vi "G#Debugger_GUI.vi"() -> ()   [LabVIEW 2017, in "G#Debugger.lvlib"]
doc: "Debugger for G# Objects."
uses:
  <vilib>/addons/_AddQ/G#Debugger/G#Debugger.lvlib
  <vilib>/addons/_AddQ/G#Object/G#Object.lvclass
  <vilib>/addons/_AddQ/G#Debugger/private/G#Debugger_DebugDialog.vi
  <vilib>/Platform/browser.llb/Open URL in Default Browser (string).vi
  <vilib>/addons/_AddQ/G#Debugger/G#Debugger_CloneUI.vi
  <vilib>/addons/_AddQ/G#Debugger/G#RemoteProxy/G#RemoteProxy.lvclass
panel:
  in  "OpClnUI":bool
  in  "RootClass":i32(ring) caption="G# Clone"
  in  "AggregatorsTags":i32(listbox)
  in  "Help":bool
  out "Application Instance":string
  in  "Window Behaviour":bool
  in  "Window Transparency":u8(slide) max=75 scale=0.0..75.0
  in  "External Create Process Running":bool
  in  "Tab Control":enum32{"Objects", "Trace", "Active Debug"}(tab)
  in  "Aggregators":i32(listbox)
  in  "AggregatesTags":i32(listbox)
  in  "Sorting":enum16{"Creation order", "By aggregation"}(ring)
  in  "Aggregates":i32(listbox)
  in  "Highlight Aggregates?":bool=TRUE
  out "To String":string
  in  "Attributes":bool
  in  "Inheritance":i32(listbox)
  in  "Destroy":bool
  in  "Object Tree":string(tree)
  in  "Refresh":bool
  out "# of Users":i32
  out "Counter":bool
  out "Ref Valid":bool
  out "Object Name":string
  out "Full Class Name":string
  in  "Poll Time (ms)":i32=200 min=0
  in  "Garbage collect":bool
  out "Object ID":u32 format="%x"
  in  "Hide Empty Classes?":bool=TRUE
  out "Owner":string
  in  "Connect":bool
  out "Connected?":bool
  in  "ShowAggregators":bool
  in  "Filter Expression":string
  in  "Trace Direction":bool=TRUE
  in  "Clear":bool
  in  "Save":bool
  out "Trace":string
  in  "Max Lines":u32=1000
  out "Run State":string
  out "CachedObjId":u32 caption="Object ID" format="%x"
  in  "Abort VI":bool
  in  "Run VI":bool
  in  "Open Panel":bool
  in  "DebugTree":string(tree)
  in  "Enable Active Debug":bool
  out "Icon":picture
  out "Cached Ref Valid":bool
  in  "Wait Until Done":bool=TRUE
  out "Cached Reference Class Name":string
  out "G# Version":string
  # "G# Debugger"
  # "These logs will also always appear in the NI LabVIEW Desktop Execution Trace, even without debugger running."
  # "The last created reference is automatically cashed and copied to all the new selected , opened or executed methods 'reference in'."
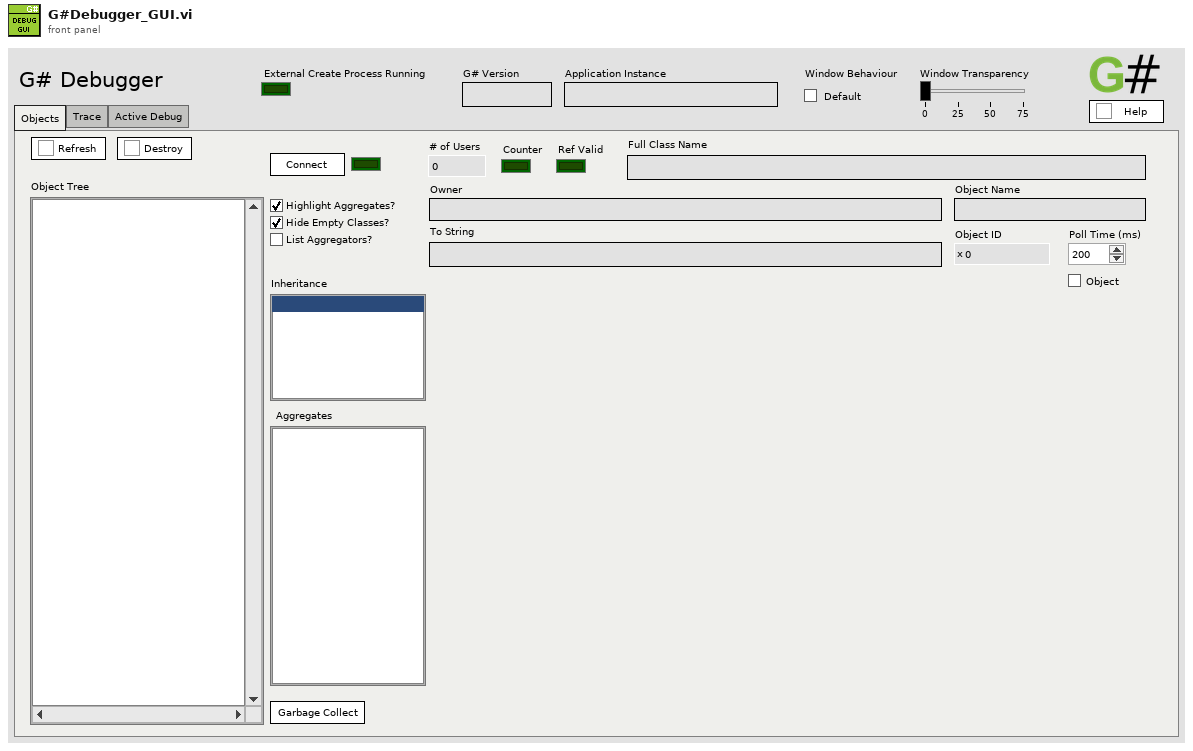
[diagram p1: front panel]
types:
  T1 = typedef "G#Debugger.lvlib/G#Debugger_Refs.ctl" = cluster{"class information dvr":refnum<data-value>, "sub panel dvr":refnum<data-value>, "GUI event":refnum<user-event>, "Active Project":refnum<vi>, "Front Panel":refnum<vi>}
  T2 = enum8{"Enabled", "Disabled", "Disabled and Grayed Out"}
  T3 = cluster{"Active Item Row Number":i32, "name":string}
  T4 = enum32{"Invalid", "Default", "Floating", "Floating/Auto-Hide", "Modal"}
  T5 = typedef "G#Debugger.lvlib/G#Debugger_SubPanelInfo.ctl" = cluster{"Ref":refnum<class "G#Object.lvclass">, "class hierarchy":T6[], "class attributes":path[], "object attributes":path[], "inheritance index":i32, "is class attributes":bool, "vi reference":refnum<vi>}
  T6 = typedef "G#Object.lvclass/G#Object_ClassHierarchy.ctl" = cluster{"ClassName":string, "FullClassName":string, "ClassPath":path, "IsLeaf":bool}
  T7 = enum32{"Bad", "Idle", "Run top level", "Running"}
  T8 = cluster{"Active Item Row Number":i32, "name":string}[]
  T9 = typedef "imagedata.ctl" = cluster{"image type":i32, "image depth":i32, "image":u8[], "mask":u8[], "colors":u32[], "Rectangle":cluster{"left":i16, "top":i16, "right":i16, "bottom":i16}}
  T10 = typedef "G#Object.lvclass/G#Object_EventType.ctl" = enum16{"Created new", "Looked up existing", "Deleted", "Forced delete", "Not deleted", "Garbage collected", "Cleared", "User", "Error", "External create object", "External create class attributes", "Created class attributes", "Run constructor", "Run constructor done", "Run open method", "Run open method done"}
  T11 = typedef "G#Object.lvclass/G#Object_ObjectInfoType.ctl" = cluster{"ObjectName":string, "ObjectID":u32, "Users":i32, "Counter":bool, "AttributeRefs":u32[], "FullClassName":string, "ClassName":string, "CreateMethod":T12, "GenericDestructorExists":bool, "Owner":string}
  T12 = typedef "G#Object.lvclass/G#Object_CreateMethod.ctl" = enum16{"Create", "Create or look up existing", "Look up existing"}
  T13 = typedef "G#Debugger.lvlib/G#Debugger_TreeElement.ctl" = cluster{"Name":string, "Tag":string, "ParentTag":string, "Position":i32}
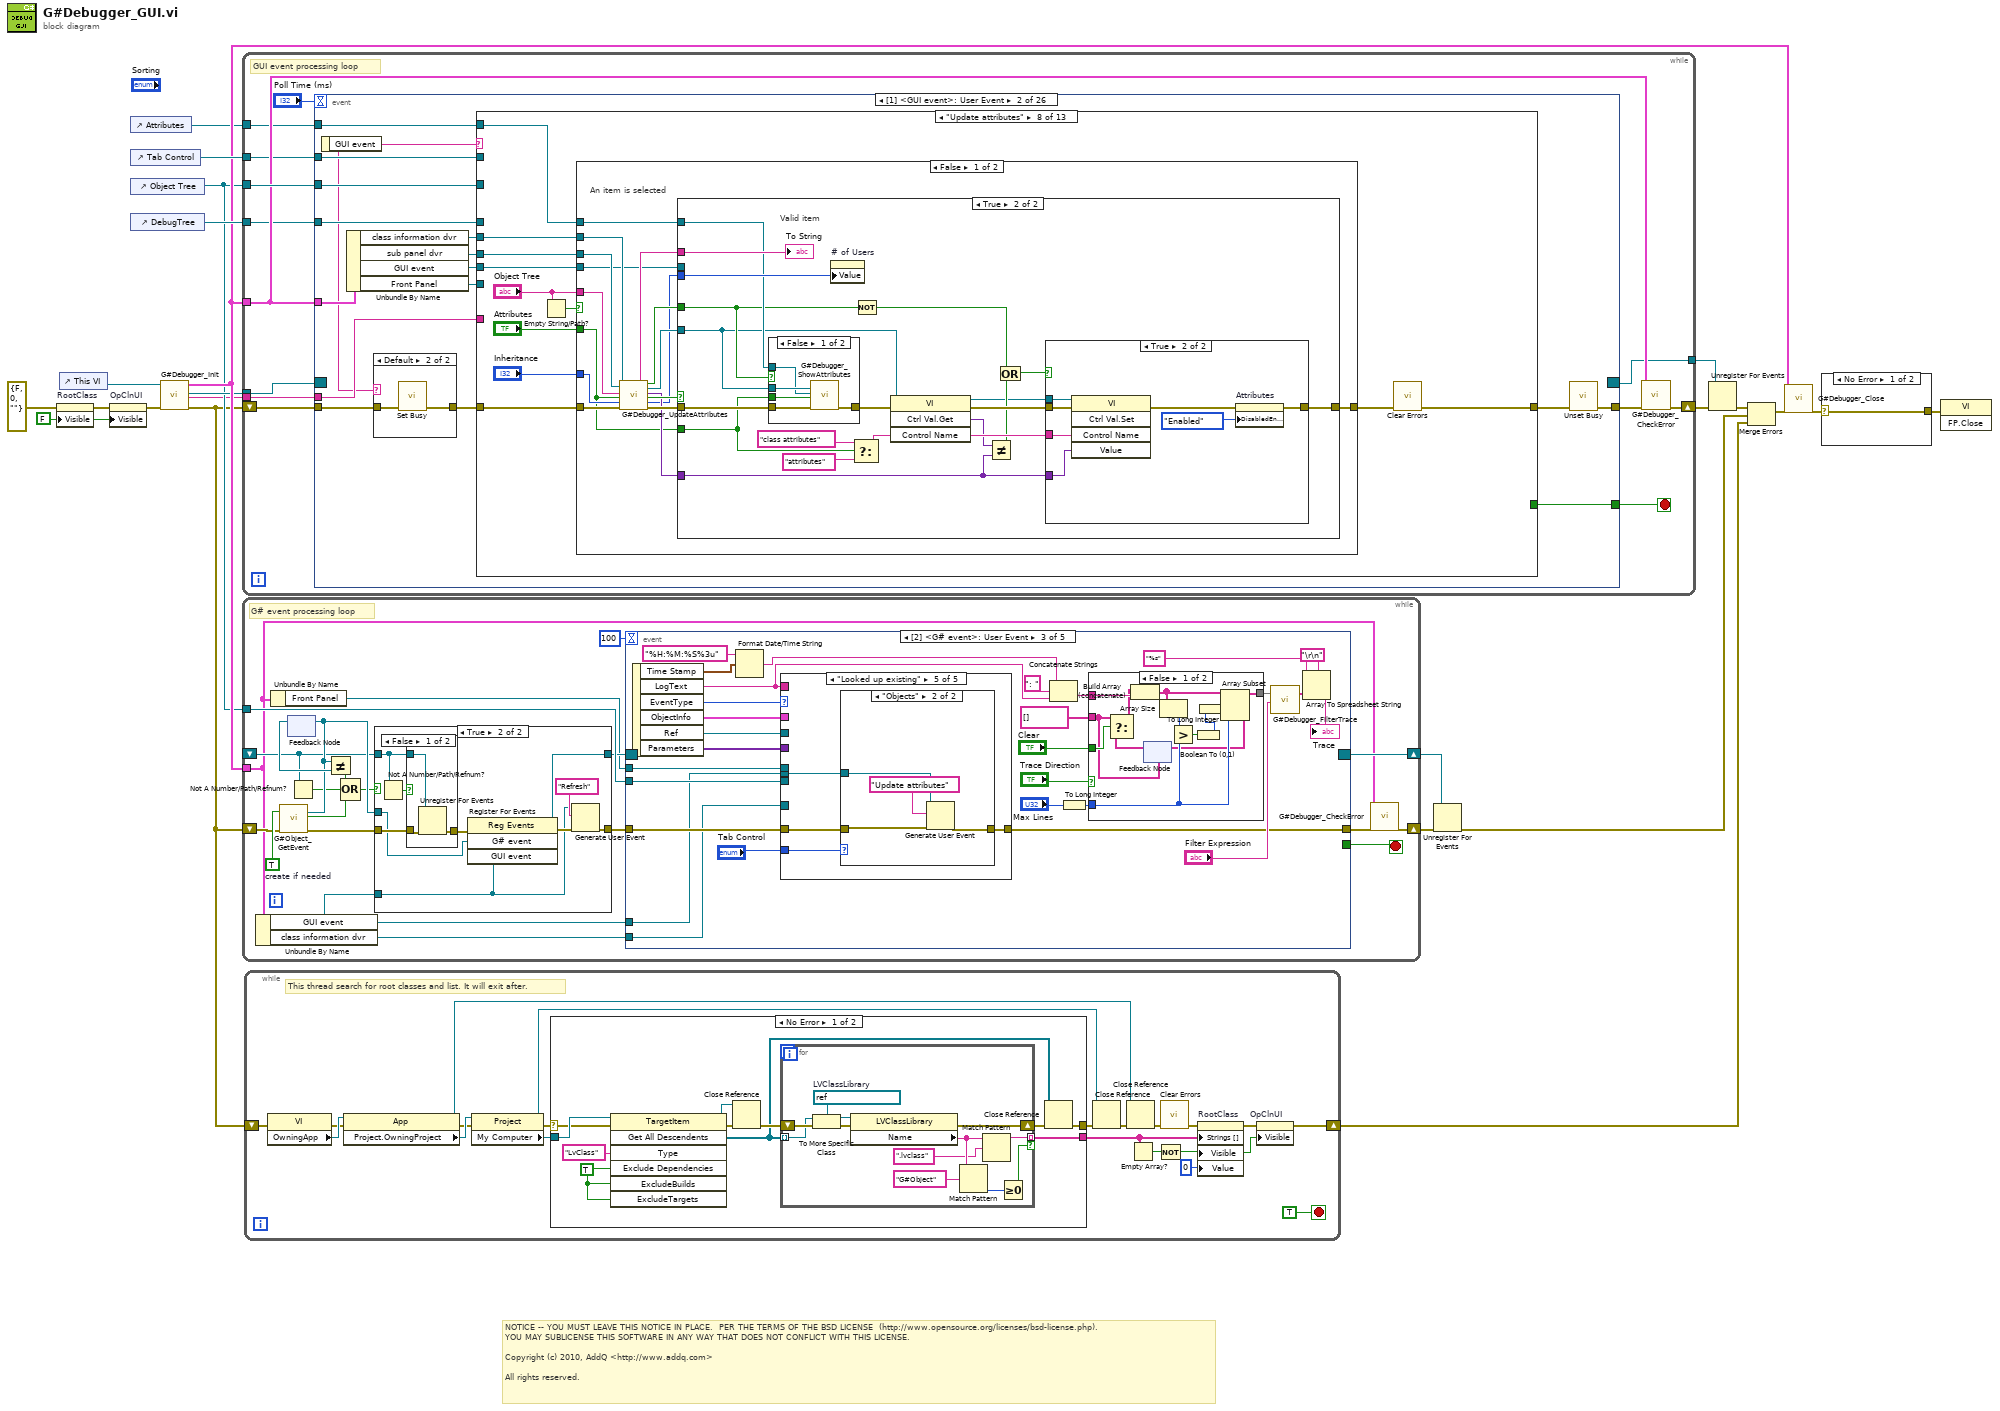
[diagram p0: block diagram]
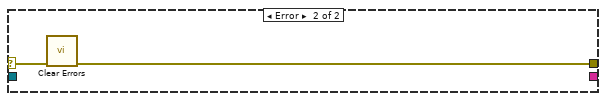
[diagram p2: hidden frame]
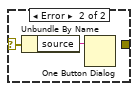
[diagram p3: hidden frame]
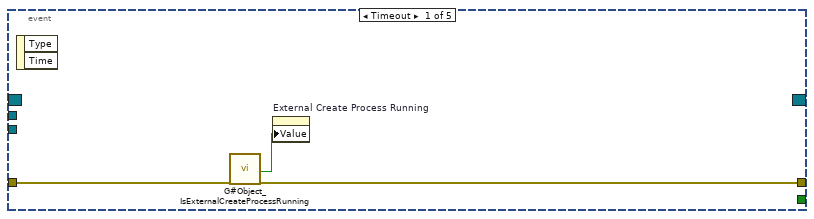
[diagram p6: hidden frame]
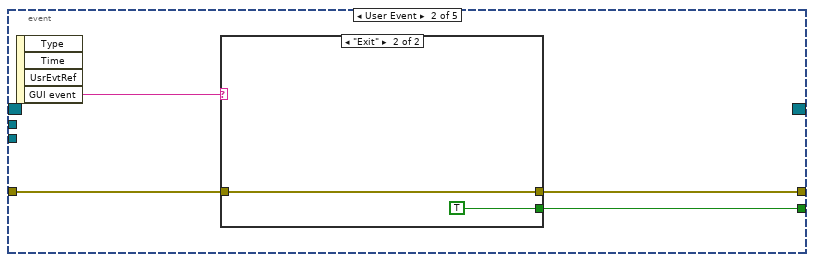
[diagram p7: hidden frame]
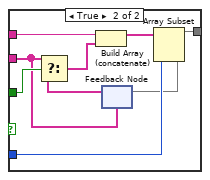
[diagram p9: hidden frame]
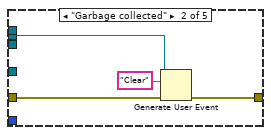
[diagram p11: hidden frame]
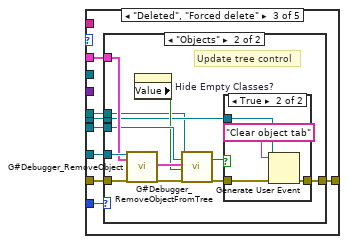
[diagram p12: hidden frame]
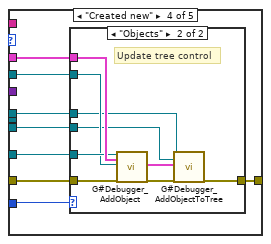
[diagram p15: hidden frame]
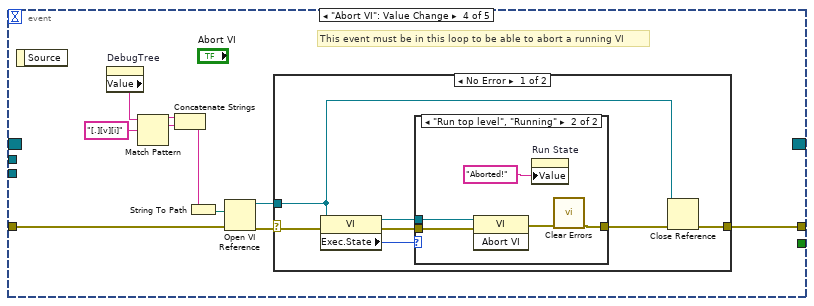
[diagram p18: hidden frame]
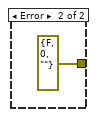
[diagram p20: hidden frame]
diagram:
  w4 = FALSE ("Visible")
  # "NOTICE -- YOU MUST LEAVE THIS NOTICE IN PLACE.  PER THE TERMS OF THE BSD LICENSE  (http://www.opensource.org/licenses/bsd-license.php).\nYOU MAY SUBLICENSE THIS SOFTWARE IN ANY WAY THAT DOES NOT CONFLICT WITH THIS LICENSE.\n\nCopyright (c) 2010, AddQ <http://www.addq.com>\n\nAll rights reserved."
  n1 = property on="RootClass" class="Ring (strict)"(error in=errorcluster {"status"=FALSE, "code"=0, "source"=""} ("error in (no error)"), "Visible"=w4) -> (error out=w3:errorcluster)  [unwired: 1 in, 1 out]
  n2 = control-ref of="This VI"() -> (w10:refnum<vi>)
  n3 = property on="OpClnUI" class="Bool"(error in=w3, "Visible"=w4) -> (error out=w1:errorcluster)  [unwired: 1 in, 1 out]
  n4 = control-ref of="Attributes"() -> (w9:refnum<vi>)
  n5 = control-ref of="Tab Control"() -> (w23:refnum<vi>)
  n6 = control-ref of="Object Tree"() -> (w12:refnum<vi>)
  n7 = control-ref of="DebugTree"() -> (w22:refnum<vi>)
  n8 = call <vilib>:"G#Debugger_Init.vi"("This VI"=w10, "error in (no error)"=w1) -> ("refs"=w21:T1, "GUI Event Registration Refnum"=w19:refnum<event-registration>, "Application Instance"=w11:string, "error out"=w6:errorcluster)  [unwired: 14 in]
  n9 = while {
    shift-right: [w34] -> w18
    shift-left: w6 -> [w29]
    tunnel: w12 -> [w36]
    tunnel: w21 -> [w32]
    tunnel: w23 -> [w31]
    tunnel: w22 -> [w30]
    tunnel: w19 -> [w28]
    tunnel: [w25] -> w17
    tunnel: w11 -> [w26]
    tunnel: w9 -> [w24]
    stop <- w35 stop-if-true
    # "GUI event processing loop"
    n10 = event shown="[1] <GUI event>: User Event" {
      selector: w28 -> [_ _ _ _ _ _ _ _ _ _ _ _ _ _ _ _ _ _ _ _ _ _ _ _ _ _]
      dyn-events: [_ _ _ _ _ _ _ _ _ _ _ _ _ _ _ _ _ _ _ _ _ _ _ _ _ _] -> w25
      timeout: "Poll Time (ms)" -> [_ _ _ _ _ _ _ _ _ _ _ _ _ _ _ _ _ _ _ _ _ _ _ _ _ _]
      tunnel: w29 -> [w42 w76 w477 w484 w494 w508 w512 w554 w589 w610 w617 w621 w628 w633 w636 w658 w683 w691 w730 w737 w740 w747 w762 w767 w788 w813]
      tunnel: [w39 w78 w477 w484 w493 w507 w511 w536 w588 w609 w618 w619 w626 w630 w640 w653 w680 w690 w729 w736 w739 w747 w761 w764 w784 w798] -> w33
      tunnel: w36 -> [_ w89 w478 w485 _ _ _ w553 _ _ w616 _ _ _ _ w652 _ _ _ _ _ _ _ w766 _ _]
      tunnel: [_ w88 _ _ _ FALSE _ _ _ _ _ _ _ _ _ _ _ _ _ _ _ _ _ _ _ _] -> w35
      tunnel: w32 -> [w46 w87 _ _ w492 w506 w510 w549 _ w608 _ w620 w627 _ w638 w649 _ w689 _ _ _ _ _ w763 _ _]
      tunnel: w31 -> [_ w84 _ _ _ _ _ _ _ _ _ _ _ _ _ _ _ _ _ _ _ _ _ _ _ _]
      tunnel: w30 -> [_ w82 _ _ _ _ _ _ _ _ _ _ _ _ _ _ _ w692 _ _ _ _ _ _ _ _]
      tunnel: w26 -> [_ w81 _ _ _ _ _ _ _ _ _ _ _ _ _ _ _ w688 _ _ _ _ _ _ _ _]
      tunnel: w24 -> [_ w74 _ _ _ _ _ _ _ _ _ _ _ _ _ _ _ _ _ _ _ _ _ _ _ _]
      event Timeout {
        # "redraw FP"
        n11 = event-data() -> ()  [unwired: 1 in, 2 out]
        n12 = Unbundle By Name(w46) -> ("Front Panel"=w40:refnum<vi>, "GUI event"=w45:refnum<user-event>)
        n13 = property on="Tab Control" class="TabCtl (strict)"(error in=w42) -> (error out=w43:errorcluster, "Value"=w44:enum32{"Objects", "Trace", "Active Debug"})  [unwired: 1 in, 1 out]
        n14 = case shown="\"Objects\"" w44 {
          tunnel: w43 -> [w47 w57 w71]
          tunnel: w45 -> [_ w53 _]
          tunnel: [w47 w54 w70] -> w41
          frame Default {
          }
          frame "Objects" {
            # "Check for dead objects, every\n5th timeout."
            n15 = Generate User Event(user event=w53, event data cluster="Update attributes" ("event data"), error in=w57) -> (error out=w55:errorcluster)  [unwired: 1 in, 1 out]
            n16 = feedback #1(u64 0) -> (w49:u64)
            n17 = Quotient & Remainder(x=w49, y=u64 5) -> (x-y*floor(x/y)=w52:u64)  [unwired: 1 out]
            n18 = Increment(x=w49) -> (x+1=w48:u64)
            n19 = feedback-in #1(w48) -> ()
            n20 = case shown="0" w52 {
              tunnel: w55 -> [w58 w63]
              tunnel: [w58 w62] -> w54
              tunnel: w53 -> [_ w61]
              frame Default {
              }
              frame 0 {
                n21 = call <vilib>:"G#Object_CleanUp.vi"("error in (no error)"=w63) -> ("any dead objects?"=w59:bool, "error out"=w60:errorcluster)  [unwired: 17 in]
                n22 = case shown="True" w59 {
                  tunnel: w60 -> [w64 w67]
                  tunnel: [w64 w66] -> w62
                  tunnel: w61 -> [_ w65]
                  frame False {
                  }
                  frame True {
                    # "Object died, refresh"
                    n23 = Generate User Event(user event=w65, event data cluster="Refresh" ("event data"), error in=w67) -> (error out=w66:errorcluster)  [unwired: 1 in, 1 out]
                  }
                }
              }
            }
          }
          frame "Active Debug" {
            w73 = FALSE  # set
            n24 = call <vilib>:"G#Debugger_CachedObject.vi"("error in (no error)"=w71, "set"=w73) -> ("not a refnum?"=w72:bool, "error out"=w70:errorcluster)  [unwired: 15 in, 1 out]
            n25 = Not(x=w72) -> (.not. x?=w69:bool)
            n26 = property on="Cached Ref Valid" class="Bool (strict)"("Value"=w69) -> ()  [unwired: 2 in, 2 out]
          }
        }
        n27 = property class="Pnl"(reference=w40, error in=w41, "DeferPanUpdts"=FALSE ("Defer Panel Updates"), "DeferPanUpdts"=TRUE ("Defer Panel Updates")) -> (error out=w39:errorcluster)  [unwired: 1 out]
      }
      event User Event {
        n28 = event-data() -> ("GUI event"=w77:string)  [unwired: 1 in]
        n29 = Unbundle By Name(w87) -> ("class information dvr"=w86:refnum<data-value>, "sub panel dvr"=w85:refnum<data-value>, "GUI event"=w83:refnum<user-event>, "Front Panel"=w80:refnum<vi>)
        n30 = case shown="Default" w77 {
          tunnel: w76 -> [w90 w92]
          tunnel: [w90 w91] -> w75
          frame "Clear object tab", "Update attributes" {
          }
          frame Default {
            n31 = call <vilib>:"Set Busy.vi"("error in (no error)"=w92) -> ("error out"=w91:errorcluster)  [unwired: 9 in, 1 out]
          }
        }
        n32 = case shown="\"Update attributes\"" w77 {
          selector: w77 -> [_ _ _ _ _ _ _ _ _ w320 _ _ w473]
          tunnel: [w93 w94 w128 w138 w145 w151 w175 w184 w276 w316 w326 w370 w474] -> w79
          tunnel: w75 -> [w93 w123 w129 w138 w144 w161 w179 w181 w277 w316 w331 w375 w474]
          tunnel: [_ _ _ _ TRUE _ _ _ _ _ _ _ _] -> w88
          tunnel: w86 -> [_ _ _ _ _ w159 w177 w187 _ _ w329 w373 _]
          tunnel: w89 -> [_ w116 _ _ _ w158 w178 _ _ _ w325 w369 _]
          tunnel: w85 -> [_ _ _ _ _ _ _ w186 _ _ _ _ _]
          tunnel: w84 -> [_ w124 _ _ _ _ _ _ _ _ _ _ _]
          tunnel: w83 -> [_ w121 w127 _ _ w150 w174 w185 _ _ _ _ _]
          tunnel: w82 -> [_ w117 _ _ _ _ _ _ _ _ _ _ _]
          tunnel: w81 -> [_ w112 _ _ _ _ _ _ _ _ _ _ _]
          tunnel: w80 -> [_ w98 _ _ _ w154 w172 _ _ _ w321 w365 _]
          tunnel: w74 -> [_ _ _ _ _ _ _ w182 _ _ _ _ _]
          frame Default {
          }
          frame "Init" {
            w95 = FALSE ("ShowAggregators")
            w99 = TRUE ("Highlight Aggregates?")
            n33 = call <vilib>:"G#Object_GetRootClassVersion.vi"("error in (no error)"=w123) -> ("version"=→"G# Version":string, "error out"=w105:errorcluster)  [unwired: 17 in]
            n34 = invoke on="Method VI Panel" class="SubPanel" method="Remove VI"(error in=w105) -> (error out=w104:errorcluster)  [unwired: 2 in, 2 out]
            n35 = call <vilib>:"G#Debugger_ClearTree.vi"("Front Panel"=w98, "Tree"=w116, "error in (no error)"=w104) -> ("error out"=w114:errorcluster)  [unwired: 16 in]
            n36 = Equal?(x=w112, y="Main Application Instance") -> (x = y?=w110:bool)
            n37 = call <vilib>:"G#Object_IsExternalCreateProcessRunning.vi"("error in (no error)"=w114) -> ("external create process running?"=w106:bool, "error out"=w113:errorcluster)  [unwired: 15 in, 2 out]
            n38 = Select(t=T2."Disabled and Grayed Out" ("Disabled"), s=w110, f=T2."Enabled" ("Disabled")) -> (s? t:f=w107:T2)
            n39 = property on="External Create Process Running" class="Bool (strict)"("Value"=w106) -> ()  [unwired: 2 in, 2 out]
            n40 = property class="TabCtl (strict)"(reference=w124, error in=w113, "Value"=enum32{"Objects", "Trace", "Active Debug"}."Objects") -> (error out=w120:errorcluster)  [unwired: 1 out]
            n41 = property on="Aggregators" class="LstBox (strict)"("Visible"=FALSE) -> ()  [unwired: 2 in, 2 out]
            n42 = property on="Enable Active Debug" class="Bool (strict)"(error in=w120, "Value"=FALSE ("Enable Active Debug"), "DisabledEnum"=w107) -> (error out=w103:errorcluster)  [unwired: 1 in, 1 out]
            n43 = property on="Aggregates" class="LstBox (strict)"("Number of Rows"=u32 16) -> ()  [unwired: 2 in, 2 out]
            n44 = call <vilib>:"G#Debugger_ClearTree.vi"("Front Panel"=w98, "Tree"=w117, "error in (no error)"=w103) -> ("error out"=w115:errorcluster)  [unwired: 16 in]
            n45 = Generate User Event(user event=w121, event data cluster="Clear controls" ("event data"), error in=w115) -> (user event out=w102:refnum<user-event>, error out=w101:errorcluster)  [unwired: 1 in]
            n46 = property on="Hide Empty Classes?" class="Bool (strict)"("Value"=w99) -> ()  [unwired: 2 in, 2 out]
            n47 = property on="Highlight Aggregates?" class="Bool (strict)"("Value"=w99) -> ()  [unwired: 2 in, 2 out]
            n48 = Generate User Event(user event=w102, event data cluster="Refresh" ("event data"), error in=w101) -> (error out=w94:errorcluster)  [unwired: 1 in, 1 out]
            n49 = property on="ShowAggregators" class="Bool (strict)"("Value"=w95) -> ()  [unwired: 2 in, 2 out]
            n50 = property on="RootClass" class="Ring (strict)"("Visible"=w95) -> ()  [unwired: 2 in, 2 out]
            n51 = property on="OpClnUI" class="Bool"("Visible"=w95) -> ()  [unwired: 2 in, 2 out]
            "Application Instance" <- w112
          }
          frame "Clear controls" {
            w130 = ""
            n52 = property on="Run State" class="Str"("Value"=w130) -> ()  [unwired: 2 in, 2 out]
            n53 = property on="Cached Reference Class Name" class="Str"("Value"=w130) -> ()  [unwired: 2 in, 2 out]
            n54 = call "Empty Picture"() -> ("empty picture"=w132:picture)
            n55 = property on="Cached Ref Valid" class="Bool (strict)"("Value"=FALSE ("Counter")) -> ()  [unwired: 2 in, 2 out]
            n56 = property on="Icon" class="Pict"("Value"=w132) -> ()  [unwired: 2 in, 2 out]
            n57 = property on="Trace" class="Str"("Value"=w130) -> ()  [unwired: 2 in, 2 out]
            n58 = property on="CachedObjId" class="DigNum (strict)"("Value"=u32 0 ("Object ID")) -> ()  [unwired: 2 in, 2 out]
            n59 = Generate User Event(user event=w127, event data cluster="Clear object tab" ("event data"), error in=w129) -> (error out=w128:errorcluster)  [unwired: 1 in, 1 out]
          }
          frame "Clear object tab" {
            w134 = 0 ("Top Row")
            w135 = string[] [] ("Item Names")
            w136 = -1 ("Inheritance")
            w137 = ""
            w141 = FALSE ("Counter")
            n60 = property on="Object Name" class="Str"("Value"=w137) -> ()  [unwired: 2 in, 2 out]
            n61 = property on="To String" class="Str"("Value"=w137) -> ()  [unwired: 2 in, 2 out]
            n62 = property on="Full Class Name" class="Str"("Value"=w137) -> ()  [unwired: 2 in, 2 out]
            n63 = property on="Owner" class="Str"("Value"=w137) -> ()  [unwired: 2 in, 2 out]
            n64 = property on="Counter" class="Bool (strict)"("Value"=w141) -> ()  [unwired: 2 in, 2 out]
            n65 = property on="Ref Valid" class="Bool (strict)"("Value"=w141) -> ()  [unwired: 2 in, 2 out]
            n66 = property on="# of Users" class="DigNum (strict)"("Value"=0 ("Nr of Users")) -> ()  [unwired: 2 in, 2 out]
            n67 = property on="Object ID" class="DigNum (strict)"("Value"=u32 0 ("Object ID")) -> ()  [unwired: 2 in, 2 out]
            n68 = property on="Aggregates" class="LstBox (strict)"("Value"=w136, "Item Names"=w135, "Top Row"=w134) -> ()  [unwired: 2 in, 2 out]
            n69 = property on="Inheritance" class="LstBox (strict)"("Value"=w136, "Item Names"=w135, "Top Row"=w134) -> ()  [unwired: 2 in, 2 out]
            n70 = property on="Aggregators" class="LstBox (strict)"("Value"=w136, "Item Names"=w135, "Top Row"=w134) -> ()  [unwired: 2 in, 2 out]
          }
          frame "Exit" {
            n71 = property on="Enable Active Debug" class="Bool (strict)"(error in=w144) -> (error out=w143:errorcluster, "Value"=w142:bool)  [unwired: 1 in, 1 out]
            n72 = case shown="True" w142 {
              tunnel: [w147 w149] -> w145
              tunnel: w143 -> [w147 w148]
              frame False {
              }
              frame True {
                n73 = call <vilib>:"GarbageCollector.vi"("error in (no error)"=w148) -> ("error out"=w149:errorcluster)  [unwired: 16 in, 2 out]
              }
            }
          }
          frame "Refresh" {
            # "Refresh tree list"
            n74 = call <vilib>:"G#Debugger_Refresh.vi"("Objects dvr"=w159, "error in (no error)"=w161) -> ("error out"=w160:errorcluster)  [unwired: 17 in]
            n75 = call <vilib>:"G#Debugger_PopulateObjectTree.vi"("Objects dvr"=w159, "Tree"=w158, "hide empty classes?"="Hide Empty Classes?", "error in (no error)"=w160, "Front Panel"=w154) -> ("error out"=w156:errorcluster)  [unwired: 14 in]
            n76 = property on="Highlight Aggregates?" class="Bool (strict)"() -> ("Value"=w155:bool)  [unwired: 2 in, 2 out]
            n77 = case shown="True" w155 {
              tunnel: [w167 w170] -> w152
              tunnel: w156 -> [w167 w169]
              tunnel: w150 -> [_ w168]
              frame False {
              }
              frame True {
                n78 = Generate User Event(user event=w168, event data cluster="Highlight aggregates" ("event data"), error in=w169) -> (error out=w170:errorcluster)  [unwired: 1 in, 1 out]
              }
            }
            n79 = property on="ShowAggregators" class="Bool (strict)"() -> ("Value"=w153:bool)  [unwired: 2 in, 2 out]
            n80 = case shown="True" w153 {
              tunnel: w152 -> [w162 w165]
              tunnel: [w162 w164] -> w151
              tunnel: w150 -> [_ w163]
              frame False {
              }
              frame True {
                n81 = Generate User Event(user event=w163, event data cluster="ListAggregators" ("event data"), error in=w165) -> (error out=w164:errorcluster)  [unwired: 1 in, 1 out]
              }
            }
          }
          frame "Clear" {
            # "Clears tree and object cache"
            n82 = call <vilib>:"G#Debugger_ClearTree.vi"("Front Panel"=w172, "Tree"=w178, "error in (no error)"=w179) -> ("error out"=w180:errorcluster)  [unwired: 16 in]
            n83 = call <vilib>:"G#Debugger_Clear.vi"("Objects dvr"=w177, "error in (no error)"=w180) -> ("error out"=w176:errorcluster)  [unwired: 17 in]
            n84 = Generate User Event(user event=w174, event data cluster="Clear object tab" ("event data"), error in=w176) -> (error out=w175:errorcluster)  [unwired: 1 in, 1 out]
          }
          frame "Update attributes" {
            n85 = Empty String/Path?(string/path="Object Tree") -> (empty?=w189:bool)
            n86 = case shown="False" w189 {
              tunnel: w181 -> [w207 w261]
              tunnel: w187 -> [w206 _]
              tunnel: w186 -> [w205 w259]
              tunnel: "Object Tree" -> [w204 _]
              tunnel: "Attributes" -> [w192 _]
              tunnel: "Inheritance" -> [w203 _]
              tunnel: [w200 w255] -> w183
              tunnel: w185 -> [w195 w254]
              tunnel: w182 -> [w193 _]
              frame False {
                # "An item is selected"
                n87 = call <vilib>:"G#Debugger_UpdateAttributes.vi"("Objects dvr"=w206, "Subpanel dvr"=w205, "tag"=w204, "class attributes"=w192, "inheritance index"=w203, "error in (no error)"=w207) -> ("string"=w196:string, "Only read attributes"=w199:bool, "attributes reference"=w198:refnum<vi>, "attributes value"=w197:variant, "valid object"=w202:bool, "# of users?"=w194:i32, "error out"=w201:errorcluster)  [unwired: 7 in]
                n88 = case shown="True" w202 {
                  tunnel: w201 -> [w215 w235]
                  tunnel: [w209 w236] -> w200
                  tunnel: w199 -> [_ w225]
                  tunnel: w198 -> [_ w221]
                  tunnel: w197 -> [_ w228]
                  tunnel: w196 -> [_ w238]
                  tunnel: w195 -> [w208 _]
                  tunnel: w194 -> [_ w237]
                  tunnel: w193 -> [_ w234]
                  tunnel: w192 -> [_ w231]
                  frame False {
                    # "Subpanel info is invalid->Clear"
                    n89 = invoke on="Attributes" class="SubPanel" method="Remove VI"(error in=w215) -> (error out=w214:errorcluster)  [unwired: 2 in, 2 out]
                    n90 = call <vilib>:"G#Object_CleanUp.vi"("error in (no error)"=w214) -> ("any dead objects?"=w212:bool, "error out"=w213:errorcluster)  [unwired: 17 in]
                    n91 = case shown="True" w212 {
                      tunnel: [w217 w219] -> w210
                      tunnel: w213 -> [w217 w219]
                      tunnel: ["Clear object tab" ("event data") "Refresh" ("event data")] -> w211
                      frame False {
                      }
                      frame True {
                      }
                    }
                    n92 = Generate User Event(user event=w208, event data cluster=w211, error in=w210) -> (error out=w209:errorcluster)  [unwired: 1 in, 1 out]
                  }
                  frame True {
                    # "Valid item"
                    n93 = case shown="False" w225 {
                      tunnel: w235 -> [w251 w252]
                      tunnel: w234 -> [w248 _]
                      tunnel: [w250 w252] -> w226
                      tunnel: w221 -> [w249 _]
                      tunnel: w231 -> [w247 _]
                      frame False {
                        n94 = call <vilib>:"G#Debugger_ShowAttributes.vi"("VIRef"=w249, "SubPanel"=w248, "ClassAttributes"=w247, "error in (no error)"=w251) -> ("error out"=w250:errorcluster)  [unwired: 14 in, 1 out]
                      }
                      frame True {
                      }
                    }
                    n95 = property on="# of Users" class="DigNum (strict)"("Value"=w237) -> ()  [unwired: 2 in, 2 out]
                    n96 = Select(t="class attributes" ("y"), s=w231, f="attributes" ("y")) -> (s? t:f=w230:string)
                    n97 = Not(x=w225) -> (.not. x?=w224:bool)
                    n98 = invoke class="VI" method="Ctrl Val.Get"(reference=w221, error in=w226, "Control Name"=w230) -> (reference out=w220:refnum<vi>, error out=w227:errorcluster, "Get Control Value Variant"=w229:variant)  [unwired: 1 in, 1 out]
                    n99 = Not Equal?(x=w229, y=w228) -> (x != y?=w223:bool)
                    n100 = Or(x=w224, y=w223) -> (x .or. y?=w222:bool)
                    n101 = case shown="True" w222 {
                      tunnel: [w239 w245] -> w236
                      tunnel: w227 -> [w239 w243]
                      tunnel: w220 -> [_ w242]
                      tunnel: w230 -> [_ w241]
                      tunnel: w228 -> [_ w240]
                      frame False {
                      }
                      frame True {
                        n102 = invoke class="VI" method="Ctrl Val.Set"(reference=w242, error in=w243, "Control Name"=w241, "Value"=w240) -> (error out=w246:errorcluster)  [unwired: 1 in, 4 out]
                        n103 = property on="Attributes" class="SubPnl"(error in=w246, "DisabledEnum"=T2."Enabled" ("Disabled")) -> (error out=w245:errorcluster)  [unwired: 1 in, 1 out]
                      }
                    }
                    "To String" <- w238
                  }
                }
              }
              frame True {
                # "No item selected in tree"
                n104 = invoke on="Attributes" class="SubPanel" method="Remove VI"(error in=w261) -> (error out=w260:errorcluster)  [unwired: 2 in, 2 out]
                n105 = in-place {
                  in-place-border: w260 -> [w266]
                  in-place-border: [w264] -> w257
                  # "Force a subpanel update!"
                  n106 = in-place-dvr #2(w259) -> (w265:T5)  [unwired: 1 out]
                  n107 = Unbundle By Name(w265) -> ("vi reference"=w262:refnum<vi>)
                  n108 = Not A Number/Path/Refnum?(number/path/refnum=w262) -> (NaN/Path/Refnum?=w263:bool)
                  n109 = case shown="False" w263 {
                    tunnel: w266 -> [w269 w270]
                    tunnel: [w268 w270] -> w264
                    tunnel: w262 -> [w267 _]
                    frame False {
                      n110 = Close Reference(reference=w267, error in (no error)=w269) -> (error out=w268:errorcluster)
                    }
                    frame True {
                    }
                  }
                  n111 = in-place-dvr #2(w265) -> (w258:errorcluster)  [unwired: 1 out]
                }
                n112 = Merge Errors(w258, w257) -> (w256:errorcluster)
                n113 = Generate User Event(user event=w254, event data cluster="Clear object tab" ("event data"), error in=w256) -> (error out=w255:errorcluster)  [unwired: 1 in, 1 out]
              }
            }
            n114 = call <vilib>:"Clear Errors.vi"("error in (no error)"=w183) -> ("error out"=w184:errorcluster)  [unwired: 5 in, 1 out]
          }
          frame "Run VI" {
            n115 = property on="DebugTree" class="Tree (strict)"() -> ("Value"=w271:string)  [unwired: 2 in, 2 out]
            n116 = Match Pattern(string=w271, regular expression="[.][v][i]") -> (before substring=w274:string, match substring=w273:string)  [unwired: 1 in, 2 out]
            n117 = Concatenate Strings(w274, w273) -> (w272:string)
            n118 = String To Path(string=w272) -> (path=w278:path)
            n119 = Open VI Reference(vi path=w278, error in (no error)=w277) -> (vi reference=w280:refnum<vi>, error out=w279:errorcluster)  [unwired: 4 in]
            n120 = case shown="No Error" w279 {
              selector: w279 -> [w285 _]
              tunnel: [w291 errorcluster {"status"=FALSE, "code"=0, "source"=""} ("error in (no error)")] -> w276
              tunnel: w280 -> [w284 _]
              tunnel: w278 -> [w289 _]
              frame No Error {
                n121 = stacked-sequence {
                  tunnel: w289 -> [w297]
                  tunnel: [w297] -> w288
                  frame #0 {
                    "Run State" <- "Running..." ("Run State")
                  }
                }
                n122 = property class="VI"(reference=w284, error in=w285) -> (error out=w282:errorcluster, "Exec.State"=w283:T7, "Exec.IsReentrant"=w286:bool)  [unwired: 1 out]
                n123 = case shown="\"Run top level\"" w283 {
                  tunnel: [FALSE TRUE w294 w295] -> w287
                  tunnel: w286 -> [_ _ w294 w295]
                  frame Default {
                  }
                  frame "Idle" {
                  }
                  frame "Run top level" {
                  }
                  frame "Running" {
                  }
                }
                n124 = case shown="True" w287 {
                  tunnel: [w303 w311] -> w290
                  tunnel: w282 -> [w303 w306]
                  tunnel: w288 -> [w302 _]
                  tunnel: [w299 w314] -> w281
                  tunnel: w283 -> [w298 _]
                  tunnel: w284 -> [_ w307]
                  frame False {
                    n125 = Strip Path(path=w302) -> (name=w301:string)  [unwired: 1 out]
                    n126 = Format Into String(format string="%s is not reentrant or in idle execution state! (%s)", w301, w298) -> (resulting string=w299:string)  [unwired: 2 in, 1 out]
                  }
                  frame True {
                    n127 = call <vilib>:"G#Debugger_RunVI.vi"("vi reference"=w307, "wait until done"="Wait Until Done", "error in (no error)"=w306) -> ("class name"=→"Cached Reference Class Name":string, "object ID"=→"CachedObjId":u32, "message"=w310:string, "not a refnum?"=w305:bool, "error out"=w311:errorcluster)  [unwired: 12 in]
                    n128 = Not(x=w305) -> (.not. x?=→"Cached Ref Valid":bool)
                    n129 = Select(t=w310, s="Wait Until Done", f="Run state is not available!") -> (s? t:f=w314:string)
                  }
                }
                n130 = property on="Run State" class="Str"("Value"=w281) -> ()  [unwired: 2 in, 2 out]
                n131 = Close Reference(reference=w284, error in (no error)=w290) -> (error out=w291:errorcluster)
              }
              frame Error {
              }
            }
          }
          frame "Wait".."Wb" {
            n132 = Decimal String To Number(string=w320, offset=5, default (0L)=u32 0 ("default (0 I32)")) -> (number=w317:u32)  [unwired: 1 out]
            n133 = Wait (ms)(milliseconds to wait=w317) -> ()  [unwired: 1 out]
          }
          frame "Highlight aggregates" {
            n134 = property on="Property Node" class="Tree (strict)"(reference=w325, error in=w331) -> (error out=w330:errorcluster, "Value"=w328:string)  [unwired: 1 out]
            n135 = call <vilib>:"G#Debugger_GetObjectFromTag.vi"("Objects dvr"=w329, "Tag"=w328, "class attributes"=FALSE, "error in (no error)"=w330) -> ("Ref"=w324:refnum<class "G#Object.lvclass">, "Found"=w322:bool, "error out"=w323:errorcluster)  [unwired: 13 in]
            n136 = case shown="True" w322 {
              tunnel: [w332 w340] -> w326
              tunnel: w325 -> [_ w352]
              tunnel: w324 -> [_ w351]
              tunnel: w323 -> [w332 w349]
              tunnel: w321 -> [_ w339]
              frame False {
              }
              frame True {
                w346 = TRUE  # remove duplicates
                # "redraw FP"
                n137 = property on="Attributes" class="Bool (strict)"(error in=w349) -> (error out=w348:errorcluster, "Value"=w347:bool)  [unwired: 1 in, 1 out]
                n138 = call <vilib>:"G#Object_GetAggregatedObjects.vi"("reference in"=w351, "class attributes (F)"=w347, "remove duplicates (F)"=w346, "error in (no error)"=w348) -> ("aggregated objects"=w345:refnum<class "G#Object.lvclass">[], "error out"=w344:errorcluster)  [unwired: 12 in, 2 out]
                n139 = for {
                  tunnel: w345 -> [w355] mode=indexing
                  shift-right: [w356] -> w350
                  shift-left: w344 -> [w358]
                  tunnel: [w357] -> w333 mode=indexing if=w353
                  n140 = call-dynamic "NotARefNum.vi"("reference in"=w355) -> ("not a refnum?"=w354:bool)  [unwired: 1 in, 1 out]
                  n141 = case shown="False" w354 {
                    tunnel: w355 -> [w363 _]
                    tunnel: w358 -> [w362 w364]
                    tunnel: [w360 _] -> w357
                    tunnel: [w359 w364] -> w356
                    frame False {
                      # "ObjectIDs are the\ntags in the object tree"
                      n142 = call-dynamic "GetObjectID.vi"("reference in"=w363, "error in (no error)"=w362) -> ("object ID"=w361:u32, "error out"=w359:errorcluster)  [unwired: 15 in, 1 out]
                      n143 = Number To Decimal String(number=w361) -> (decimal integer string=w360:string)  [unwired: 1 in]
                    }
                    frame True {
                    }
                  }
                  n144 = Not(x=w354) -> (.not. x?=w353:bool)
                }
                n145 = control-ref of="Aggregates"() -> (w338:refnum<vi>)
                n146 = control-ref of="AggregatesTags"() -> (w337:refnum<vi>)
                n147 = Array Size(array=w333) -> (size(s)=w336:i32)
                n148 = call <vilib>:"G#Debugger_Highlight.vi"("Tree"=w352, "Aggregates"=w338, "ObjectIDs"=w333, "error in (no error)"=w350, "AggregatesTags"=w337) -> ("error out"=w341:errorcluster)  [unwired: 14 in]
                n149 = Greater Or Equal?(x=w336, y=8) -> (x >= y?=w335:bool)
                n150 = property class="Pnl"(reference=w339, error in=w341, "DeferPanUpdts"=FALSE ("Defer Panel Updates"), "DeferPanUpdts"=TRUE ("Defer Panel Updates")) -> (error out=w340:errorcluster)  [unwired: 1 out]
                n151 = property on="Aggregates" class="LstBox (strict)"("Scrollbar Visible"=w335) -> ()  [unwired: 2 in, 2 out]
              }
            }
          }
          frame "ListAggregators" {
            n152 = property on="Property Node" class="Tree (strict)"(reference=w369, error in=w375) -> (error out=w374:errorcluster, "Value"=w372:string)  [unwired: 1 out]
            n153 = call <vilib>:"G#Debugger_GetObjectFromTag.vi"("Objects dvr"=w373, "Tag"=w372, "class attributes"=FALSE, "error in (no error)"=w374) -> ("Ref"=w368:refnum<class "G#Object.lvclass">, "Found"=w366:bool, "error out"=w367:errorcluster)  [unwired: 13 in]
            n154 = case shown="True" w366 {
              tunnel: [w376 w396] -> w370
              tunnel: w369 -> [_ _]
              tunnel: w368 -> [_ w395]
              tunnel: w367 -> [w376 w401]
              tunnel: w365 -> [_ w381]
              frame False {
              }
              frame True {
                # "redraw FP"
                n155 = call-dynamic "GetObjectID.vi"("reference in"=w395) -> ("object ID"=w378:u32)  [unwired: 16 in, 2 out]
                n156 = property on="Attributes" class="Bool (strict)"(error in=w401) -> (error out=w400:errorcluster, "Value"=w399:bool)  [unwired: 1 in, 1 out]
                n157 = Equal To 0?(x=w378) -> (x = 0?=w377:bool)
                n158 = case shown="False" w377 {
                  tunnel: w400 -> [w413 w464]
                  tunnel: w399 -> [w412 _]
                  tunnel: w378 -> [w406 _]
                  tunnel: [w405 w464] -> w394
                  tunnel: [w403 _] -> w387
                  tunnel: [w402 _] -> w385
                  frame False {
                    w411 = TRUE  # remove duplicates
                    n159 = call <vilib>:"G#Object_GetAllObjects.vi"("only refs (F)"=TRUE) -> ("all refs"=w408:refnum<class "G#Object.lvclass">[])  [unwired: 15 in, 3 out]
                    n160 = for {
                      tunnel: w412 -> [w420]
                      tunnel: w411 -> [w419]
                      tunnel: [w417] -> w410 mode=indexing if=w414
                      shift-right: [w418] -> w409
                      shift-left: w413 -> [w421]
                      tunnel: w408 -> [w416] mode=indexing
                      tunnel: [w416] -> w404 mode=indexing if=w414
                      n161 = call-dynamic "NotARefNum.vi"("reference in"=w416) -> ("not a refnum?"=w415:bool)  [unwired: 1 in, 1 out]
                      n162 = Not(x=w415) -> (.not. x?=w414:bool)
                      n163 = case shown="False" w415 {
                        tunnel: w421 -> [w428 w433]
                        tunnel: w420 -> [w427 _]
                        tunnel: w419 -> [w426 _]
                        tunnel: [w425 w433] -> w418
                        tunnel: w416 -> [w424 _]
                        tunnel: [w422 _] -> w417
                        frame False {
                          n164 = call <vilib>:"G#Object_GetAggregatedObjects.vi"("reference in"=w424, "class attributes (F)"=w427, "remove duplicates (F)"=w426, "error in (no error)"=w428) -> ("aggregated objects"=w423:refnum<class "G#Object.lvclass">[], "error out"=w425:errorcluster)  [unwired: 12 in, 2 out]
                          n165 = for {
                            tunnel: w423 -> [w432] mode=indexing
                            tunnel: [w431] -> w422 mode=indexing if=w429
                            n166 = call-dynamic "NotARefNum.vi"("reference in"=w432) -> ("not a refnum?"=w430:bool, "reference out"=w431:refnum<class "G#Object.lvclass">)  [unwired: 1 in]
                            n167 = Not(x=w430) -> (.not. x?=w429:bool)
                          }
                        }
                        frame True {
                        }
                      }
                    }
                    n168 = for {
                      tunnel: w410 -> [w444] mode=indexing
                      shift-right: [w440] -> w405
                      shift-left: w409 -> [w443]
                      tunnel: [w436] -> w403 mode=indexing if=w434
                      tunnel: w406 -> [w442]
                      tunnel: w404 -> [w439] mode=indexing
                      tunnel: [w435] -> w402 mode=indexing if=w434
                      # "ObjectIDs are the\ntags in the object tree"
                      n169 = for {
                        tunnel: w444 -> [w455] mode=indexing
                        tunnel: w442 -> [w453]
                        tunnel: [w450] -> w434
                        shift-right: [w451] -> w441
                        shift-left: w443 -> [w454]
                        stop <- w450 stop-if-true
                        n170 = call-dynamic "GetObjectID.vi"("reference in"=w455, "error in (no error)"=w454) -> ("object ID"=w452:u32, "error out"=w451:errorcluster)  [unwired: 15 in, 1 out]
                        n171 = Equal?(x=w453, y=w452) -> (x = y?=w450:bool)
                      }
                      n172 = case shown="True" w434 {
                        tunnel: w441 -> [w456 w463]
                        tunnel: [w456 w462] -> w440
                        tunnel: w439 -> [_ w458]
                        tunnel: [_ w460] -> w438
                        tunnel: [_ w459] -> w437
                        tunnel: [_ w457] -> w435
                        frame False {
                        }
                        frame True {
                          n173 = call-dynamic "GetObjectID.vi"("reference in"=w458) -> ("object ID"=w457:u32)  [unwired: 16 in, 2 out]
                          n174 = call-dynamic "GetObjectStatus.vi"("reference in"=w458, "simple info (F)"=TRUE, "error in (no error)"=w463) -> ("class name"=w460:string, "object name"=w459:string, "error out"=w462:errorcluster)  [unwired: 5 in, 9 out]
                        }
                      }
                      n175 = disable-structure shown="Enabled" {
                        disable-tunnel: w438 -> [w448 _]
                        disable-tunnel: w437 -> [w447 w449]
                        disable-tunnel: [w445 w449] -> w436
                        frame Enabled {
                          n176 = Format Into String(format string="%s:%s", w448, w447) -> (resulting string=w445:string)  [unwired: 2 in, 1 out]
                        }
                        frame Disabled {
                        }
                      }
                    }
                  }
                  frame True {
                  }
                }
                n177 = for {
                  tunnel: w385 -> [w469] mode=indexing
                  tunnel: w387 -> [w470] mode=indexing
                  tunnel: [w468] -> w389 mode=indexing
                  n178 = Bundle(cluster=T3 {"Active Item Row Number"=0, "name"=""}, "Active Item Row Number"=w469, "name"=w470) -> (w468:T3)
                }
                n179 = Sort 1D Array(array=w385) -> (sorted array=w384:u32[])
                n180 = Array Size(array=w384) -> (size(s)=w392:i32)
                n181 = Greater Or Equal?(x=w392, y=7) -> (x >= y?=w391:bool)
                n182 = Number To Decimal String(number=w384) -> (decimal integer string=w382:string[])  [unwired: 1 in]
                n183 = property on="Aggregators" class="LstBox (strict)"("Scrollbar Visible"=w391) -> ()  [unwired: 2 in, 2 out]
                n184 = Sort 1D Array(array=w389) -> (sorted array=w388:T8)
                n185 = for {
                  tunnel: w388 -> [w466] mode=indexing
                  tunnel: [w465] -> w386 mode=indexing
                  n186 = Unbundle By Name(w466) -> ("name"=w465:string)
                }
                n187 = property on="Aggregators" class="LstBox (strict)"(error in=w394, "Item Names"=w386) -> (error out=w393:errorcluster)  [unwired: 1 in, 1 out]
                n188 = control-ref of="AggregatorsTags"() -> (w390:refnum<vi>)
                n189 = property on="Property Node" class="LstBox (strict)"(reference=w390, "Item Names"=w382, "Value"=-1, "Top Row"=0) -> ()  [unwired: 1 in, 2 out]
                n190 = property class="Pnl"(reference=w381, error in=w393, "DeferPanUpdts"=FALSE ("Defer Panel Updates"), "DeferPanUpdts"=TRUE ("Defer Panel Updates")) -> (error out=w396:errorcluster)  [unwired: 1 out]
              }
            }
          }
          frame "Connected", "Disconnected" {
            n191 = Equal?(x=w473, y="Connected") -> (x = y?=→"Connected?":bool)
          }
        }
        n192 = call <vilib>:"Unset Busy.vi"("error in (no error)"=w79) -> ("error out"=w78:errorcluster)  [unwired: 10 in]
      }
      event "Aggregates": Double Click {
        n193 = event-data() -> ()  [unwired: 1 in, 1 out]
        n194 = control-ref of="AggregatesTags"() -> (w476:refnum<vi>)
        n195 = control-ref of="Aggregates"() -> (w475:refnum<vi>)
        n196 = property class="LstBox (strict)"(reference=w476) -> ("Item Names"=w480:string[])  [unwired: 1 in, 2 out]
        n197 = property class="LstBox (strict)"(reference=w475) -> ("Value"=w481:i32)  [unwired: 1 in, 2 out]
        n198 = Index Array(array=w480, index=w481) -> (element=w479:string)
        n199 = property class="Tree (strict)"(reference=w478, "Val(Sgnl)"=w479) -> ()  [unwired: 1 in, 2 out]
      }
      event "Aggregators": Double Click {
        n200 = event-data() -> ()  [unwired: 1 in, 1 out]
        n201 = control-ref of="AggregatorsTags"() -> (w483:refnum<vi>)
        n202 = control-ref of="Aggregators"() -> (w482:refnum<vi>)
        n203 = property class="LstBox (strict)"(reference=w482) -> ("Value"=w488:i32)  [unwired: 1 in, 2 out]
        n204 = property class="LstBox (strict)"(reference=w483) -> ("Item Names"=w487:string[])  [unwired: 1 in, 2 out]
        n205 = Index Array(array=w487, index=w488) -> (element=w486:string)
        n206 = property class="Tree (strict)"(reference=w485, "Val(Sgnl)"=w486) -> ()  [unwired: 1 in, 2 out]
      }
      event "ShowAggregators": Value Change {
        n207 = event-data() -> ("NewVal"=w490:bool)  [unwired: 1 in]
        n208 = Unbundle By Name(w492) -> ("GUI event"=w491:refnum<user-event>)
        n209 = property on="Aggregators" class="LstBox (strict)"("Visible"=w490) -> ()  [unwired: 2 in, 2 out]
        n210 = case shown="False" w490 {
          tunnel: w494 -> [w496 w500]
          tunnel: [w496 w499] -> w493
          tunnel: w491 -> [_ w498]
          tunnel: [u32 16 ("Number of Rows") u32 7 ("Number of Rows")] -> w489
          frame False {
          }
          frame True {
            n211 = Generate User Event(user event=w498, event data cluster="ListAggregators" ("event data"), error in=w500) -> (error out=w499:errorcluster)  [unwired: 1 in, 1 out]
          }
        }
        n212 = property on="Aggregates" class="LstBox (strict)"("Number of Rows"=w489) -> ()  [unwired: 2 in, 2 out]
      }
      event Panel Close? {
        n213 = event-data() -> ()  [unwired: 1 in, 3 out]
        n214 = Unbundle By Name(w506) -> ("GUI event"=w503:refnum<user-event>)
        n215 = Generate User Event(user event=w503, event data cluster="Exit" ("event data"), error in=w508) -> (error out=w507:errorcluster)  [unwired: 1 in, 1 out]
        n216 = event-data("Discard?"=TRUE) -> ()  [unwired: 1 in, 1 out]
      }
      event "Tab Control": Value Change {
        n217 = event-data() -> ("NewVal"=w513:enum32{"Objects", "Trace", "Active Debug"})  [unwired: 1 in, 4 out]
        n218 = Unbundle By Name(w510) -> ("GUI event"=w509:refnum<user-event>)
        n219 = case shown="\"Objects\"" w513 {
          tunnel: w512 -> [w517 w520]
          tunnel: [w519 w520] -> w511
          tunnel: w509 -> [w515 _]
          frame "Objects" {
            # "Refresh tree control"
            n220 = Generate User Event(user event=w515, event data cluster="Clear object tab" ("event data"), error in=w517) -> (error out=w516:errorcluster)  [unwired: 1 in, 1 out]
            n221 = Generate User Event(user event=w515, event data cluster="Refresh" ("event data"), error in=w516) -> (error out=w519:errorcluster)  [unwired: 1 in, 1 out]
          }
          frame Default {
          }
        }
      }
      event "Object Tree": Value Change {
        w565 = TRUE  # simple info
        n222 = event-data() -> ()  [unwired: 1 in, 1 out]
        n223 = property class="Tree (strict)"(reference=w553, error in=w554) -> (error out=w535:errorcluster, "Value"=w552:string)  [unwired: 1 out]
        n224 = Unbundle By Name(w549) -> ("class information dvr"=w548:refnum<data-value>, "GUI event"=w530:refnum<user-event>)
        n225 = property on="Attributes" class="Bool (strict)"(error in=w535) -> (error out=w534:errorcluster, "Value"=w533:bool)  [unwired: 1 in, 1 out]
        n226 = call <vilib>:"G#Debugger_GetObjectFromTag.vi"("Objects dvr"=w548, "Tag"=w552, "class attributes"=w533, "error in (no error)"=w534) -> ("Ref"=w559:refnum<class "G#Object.lvclass">, "error out"=w566:errorcluster)  [unwired: 13 in, 1 out]
        n227 = call-dynamic "GetObjectStatus.vi"("reference in"=w559, "simple info (F)"=w565, "error in (no error)"=w566) -> ("full class name"=→"Full Class Name":string, "# of users?"=→"# of Users":i32, "class name"=w537:string, "reference out"=w557:refnum<class "G#Object.lvclass">, "not a refnum?"=w562:bool, "object name"=→"Object Name":string, "counter?"=→"Counter":bool, "error out"=w558:errorcluster)  [unwired: 5 in, 4 out]
        n228 = Not(x=w562) -> (.not. x?=→"Ref Valid":bool)
        n229 = property on="Cached Reference Class Name" class="Str"("Value"=w537) -> ()  [unwired: 2 in, 2 out]
        n230 = call <vilib>:"G#Object_GetClassHierarchy.vi"("reference in"=w557, "error in (no error)"=w558) -> ("reference out"=w546:refnum<class "G#Object.lvclass">, "class hierarchy"=w556:T6[], "error out"=w547:errorcluster)  [unwired: 15 in]
        n231 = call-dynamic "GetObjectID.vi"("reference in"=w546, "error in (no error)"=w547) -> ("reference out"=w542:refnum<class "G#Object.lvclass">, "object ID"=w538:u32, "error out"=w543:errorcluster)  [unwired: 15 in]
        "Object ID" <- w538
        n232 = property on="CachedObjId" class="DigNum (strict)"("Value"=w538) -> ()  [unwired: 2 in, 2 out]
        n233 = for {
          tunnel: w556 -> [w578] mode=indexing
          tunnel: [w577] -> w551 mode=indexing
          n234 = Unbundle By Name(w578) -> ("ClassName"=w577:string)
        }
        n235 = call-dynamic "G#Object_GetOwner.vi"("reference in"=w542, "error in (no error)"=w543) -> ("reference out"=w540:refnum<class "G#Object.lvclass">, "owner"=→"Owner":string, "error out"=w541:errorcluster)  [unwired: 15 in]
        n236 = call <vilib>:"G#Debugger_CachedObject.vi"("cached object"=w540, "error in (no error)"=w541, "set"=TRUE) -> ("error out"=w532:errorcluster)  [unwired: 14 in, 2 out]
        n237 = case shown="True" "Highlight Aggregates?" {
          tunnel: w532 -> [w572 w576]
          tunnel: [w572 w575] -> w531
          tunnel: w530 -> [_ w573]
          frame False {
          }
          frame True {
            n238 = Generate User Event(user event=w573, event data cluster="Highlight aggregates" ("event data"), error in=w576) -> (error out=w575:errorcluster)  [unwired: 1 in, 1 out]
          }
        }
        n239 = Array Size(array=w551) -> (size(s)=w522:i32)
        n240 = Decrement(x=w522) -> (x-1=w550:i32)
        n241 = property on="Inheritance" class="LstBox (strict)"("Item Names"=w551, "Value"=w550, "Top Row"=0) -> ()  [unwired: 2 in, 2 out]
        n242 = Generate User Event(user event=w530, event data cluster="Update attributes" ("event data"), error in=w531) -> (user event out=w526:refnum<user-event>, error out=w528:errorcluster)  [unwired: 1 in]
        n243 = Greater Or Equal?(x=w522, y=8) -> (x >= y?=w524:bool)
        n244 = case shown="True" "ShowAggregators" {
          tunnel: w528 -> [w567 w570]
          tunnel: [w567 w569] -> w527
          tunnel: w526 -> [_ w568]
          frame False {
          }
          frame True {
            n245 = Generate User Event(user event=w568, event data cluster="ListAggregators" ("event data"), error in=w570) -> (error out=w569:errorcluster)  [unwired: 1 in, 1 out]
          }
        }
        n246 = property on="Inheritance" class="LstBox (strict)"("Scrollbar Visible"=w524) -> ()  [unwired: 2 in, 2 out]
        n247 = call <vilib>:"Clear Errors.vi"("error in (no error)"=w527) -> ("error out"=w536:errorcluster)  [unwired: 5 in, 1 out]
      }
      event "DebugTree": Value Change {
        n248 = event-data() -> ("NewVal"=w583:string)  [unwired: 1 in, 4 out]
        n249 = Match Pattern(string=w583, regular expression="[.][v][i]") -> (before substring=w581:string, match substring=w580:string)  [unwired: 1 in, 2 out]
        n250 = Concatenate Strings(w581, w580) -> (w579:string)
        n251 = String To Path(string=w579) -> (path=w584:path)
        n252 = Open VI Reference(vi path=w584, error in (no error)=w589) -> (vi reference=w587:refnum<vi>, error out=w586:errorcluster)  [unwired: 4 in]
        n253 = case shown="No Error" w586 {
          selector: w586 -> [w593 _]
          tunnel: [w596 w606] -> w588
          tunnel: w587 -> [w591 _]
          tunnel: [w594 w607] -> w585
          frame No Error {
            n254 = call <vilib>:"G#Debugger_SetCachedRef.vi"("MethodVIref"=w591, "error in (no error)"=w593) -> ("error out"=w592:errorcluster)  [unwired: 17 in]
            n255 = invoke on="Method VI Panel" class="SubPanel" method="Insert VI"(error in=w592, "VI Ref"=w591) -> (error out=w590:errorcluster)  [unwired: 2 in, 3 out]
            n256 = case shown="No Error" w590 {
              selector: w590 -> [w600 _]
              tunnel: [w599 w602] -> w595
              tunnel: w591 -> [w601 _]
              tunnel: [w597 w604] -> w594
              frame No Error {
                n257 = invoke class="VI" method="VI Icon.Get as Image Data"(reference=w601, error in=w600) -> (error out=w599:errorcluster, "ImageData"=w598:T9)  [unwired: 4 in, 4 out]
                n258 = call <vilib>:"Draw Flattened Pixmap.vi"("image data"=w598) -> ("new picture"=w597:picture)  [unwired: 8 in]
              }
              frame Error {
                n259 = vi-ref "G#Debugger.lvlib:G#Debugger_DebugDialog.vi"() -> (w603:refnum<vi>)
                n260 = invoke on="Method VI Panel" class="SubPanel" method="Insert VI"("VI Ref"=w603) -> (error out=w602:errorcluster)  [unwired: 3 in, 3 out]
                n261 = call "Empty Picture"() -> ("empty picture"=w604:picture)
              }
            }
            n262 = Close Reference(reference=w591, error in (no error)=w595) -> (error out=w596:errorcluster)
          }
          frame Error {
            n263 = invoke on="Method VI Panel" class="SubPanel" method="Remove VI"(error in=errorcluster {"status"=FALSE, "code"=0, "source"=""} ("error in (no error)")) -> (error out=w606:errorcluster)  [unwired: 2 in, 2 out]
            n264 = call "Empty Picture"() -> ("empty picture"=w607:picture)
          }
        }
        "Icon" <- w585
      }
      event "Run VI": Value Change {
        # "We need to fire a new event so we don't lock up the UI event."
        n265 = event-data() -> ()  [unwired: 1 in, 5 out]
        n266 = Unbundle By Name(w608) -> ("GUI event"=w611:refnum<user-event>)
        n267 = Generate User Event(user event=w611, event data cluster="Run VI" ("event data"), error in=w610) -> (error out=w609:errorcluster)  [unwired: 1 in, 1 out]
      }
      event "Attributes": Value Change {
        n268 = event-data() -> ()  [unwired: 1 in, 5 out]
        n269 = property class="Tree (strict)"(reference=w616, error in=w617) -> (reference out=w614:refnum<vi>, error out=w615:errorcluster, "Value"=w613:string)
        n270 = property class="Tree (strict)"(reference=w614, error in=w615, "Val(Sgnl)"=w613) -> (error out=w618:errorcluster)  [unwired: 1 out]
      }
      event "Inheritance": Value Change {
        n271 = event-data() -> ()  [unwired: 1 in, 5 out]
        n272 = Unbundle By Name(w620) -> ("GUI event"=w622:refnum<user-event>)
        n273 = Generate User Event(user event=w622, event data cluster="Update attributes" ("event data"), error in=w621) -> (error out=w619:errorcluster)  [unwired: 1 in, 1 out]
      }
      event "Refresh", "Hide Empty Classes?": Value Change {
        n274 = event-data() -> ()  [unwired: 1 in, 5 out]
        n275 = Unbundle By Name(w627) -> ("GUI event"=w624:refnum<user-event>)
        n276 = Generate User Event(user event=w624, event data cluster="Refresh" ("event data"), error in=w628) -> (error out=w626:errorcluster)  [unwired: 1 in, 1 out]
      }
      event "Clear": Value Change {
        n277 = event-data() -> ()  [unwired: 1 in, 5 out]
        n278 = call <vilib>:"G#Object_SendUserEvent.vi"("text"="Debugger clearing display!" ("Text"), "error in (no error)"=w633) -> ("error out"=w631:errorcluster)  [unwired: 16 in, 1 out]
        n279 = property on="Trace" class="Str"(error in=w631, "Value"="") -> (error out=w630:errorcluster)  [unwired: 1 in, 1 out]
      }
      event "Garbage collect": Value Change {
        n280 = event-data() -> ()  [unwired: 1 in, 5 out]
        n281 = Unbundle By Name(w638) -> ("GUI event"=w637:refnum<user-event>)
        n282 = call <vilib>:"G#Object_SendUserEvent.vi"("text"="Debugger garbage collected!" ("Text"), "error in (no error)"=w636) -> ("error out"=w644:errorcluster)  [unwired: 16 in, 1 out]
        n283 = call <vilib>:"GarbageCollector.vi"("only from same owner as caller? (T)"=FALSE, "error in (no error)"=w644) -> ("error out"=w635:errorcluster)  [unwired: 15 in, 2 out]
        n284 = call <vilib>:"Clear Errors.vi"("error in (no error)"=w635) -> ("error out"=w634:errorcluster)  [unwired: 5 in, 1 out]
        n285 = property on="Enable Active Debug" class="Bool (strict)"() -> ("Value"=w643:bool)  [unwired: 2 in, 2 out]
        n286 = case shown="True" w643 {
          tunnel: w634 -> [w646 w648]
          tunnel: [w646 w647] -> w639
          frame False {
          }
          frame True {
            n287 = call <vilib>:"G#Object_StartExternalCreateProcess.vi"("error in (no error)"=w648) -> ("error out"=w647:errorcluster)  [unwired: 18 in]
          }
        }
        n288 = property on="External Create Process Running" class="Bool (strict)"("Value"=w643) -> ()  [unwired: 2 in, 2 out]
        n289 = Generate User Event(user event=w637, event data cluster="Clear" ("event data"), error in=w639) -> (error out=w640:errorcluster)  [unwired: 1 in, 1 out]
      }
      event "Destroy": Value Change {
        n290 = event-data() -> ()  [unwired: 1 in, 5 out]
        n291 = Unbundle By Name(w649) -> ("class information dvr"=w650:refnum<data-value>)
        n292 = property class="Tree (strict)"(reference=w652, error in=w658) -> (error out=w657:errorcluster, "Value"=w651:string)  [unwired: 1 out]
        n293 = call <vilib>:"G#Debugger_GetObjectFromTag.vi"("Objects dvr"=w650, "Tag"=w651, "error in (no error)"=w657) -> ("Ref"=w654:refnum<class "G#Object.lvclass">, "Found"=w655:bool, "error out"=w656:errorcluster)  [unwired: 14 in]
        n294 = case shown="True" w655 {
          tunnel: w656 -> [w659 w665]
          tunnel: w654 -> [_ w667]
          tunnel: [w659 w666] -> w653
          tunnel: w652 -> [_ w664]
          tunnel: w651 -> [_ w663]
          frame False {
          }
          frame True {
            w669 = TRUE  # Simple Info
            n295 = call <vilib>:"G#Debugger_NavigateToPreviousTreeItem.vi"("Tree"=w664, "Tag"=w663, "error in (no error)"=w665) -> ("error out"=w662:errorcluster)  [unwired: 16 in]
            n296 = call <vilib>:"G#Object_SendUserEvent.vi"("text"="Debugger killed object!" ("Text"), "error in (no error)"=w662) -> ("error out"=w661:errorcluster)  [unwired: 16 in, 1 out]
            n297 = call-dynamic "GetObjectStatus.vi"("reference in"=w667, "simple info (F)"=w669, "error in (no error)"=w661) -> ("# of users?"=w668:i32, "error out"=w670:errorcluster)  [unwired: 5 in, 10 out]
            n298 = for {
              N: w668 -> [_]
              tunnel: [w671] -> w666
              tunnel: w670 -> [w674]
              tunnel: w667 -> [w673]
              # "Loop users"
              n299 = call-dynamic "NotARefNum.vi"("reference in"=w673) -> ("not a refnum?"=w672:bool)  [unwired: 1 in, 1 out]
              n300 = case shown="False" w672 {
                tunnel: [w676 w679] -> w671
                tunnel: w674 -> [w678 w679]
                tunnel: w673 -> [w677 _]
                frame False {
                  n301 = call-dynamic "Destroy.vi"("reference in"=w677, "error in (no error)"=w678) -> ("error out"=w675:errorcluster)  [unwired: 16 in, 1 out]
                  n302 = call <vilib>:"Clear Errors.vi"("error in (no error)"=w675) -> ("error out"=w676:errorcluster)  [unwired: 5 in, 1 out]
                }
                frame True {
                }
              }
            }
          }
        }
      }
      event "Save": Value Change {
        n303 = event-data() -> ()  [unwired: 1 in, 5 out]
        n304 = property on="Trace" class="Str"() -> ("Value"=w682:string)  [unwired: 2 in, 2 out]
        n305 = Write to Text File(text=w682, error in=w683) -> (error out=w681:errorcluster)  [unwired: 2 in, 2 out]
        n306 = call <vilib>:"Clear Errors.vi"("error in (no error)"=w681) -> ("error out"=w680:errorcluster)  [unwired: 5 in, 1 out]
      }
      event "Enable Active Debug": Value Change {
        n307 = event-data() -> ("NewVal"=w684:bool)  [unwired: 1 in, 4 out]
        n308 = Select(t="Debugger enabled active debug!" ("Text"), s=w684, f="Debugger disabled active debug!" ("Text")) -> (s? t:f=w695:string)
        n309 = call <vilib>:"G#Object_SendUserEvent.vi"("text"=w695, "error in (no error)"=w691) -> ("error out"=w687:errorcluster)  [unwired: 16 in, 1 out]
        n310 = call <vilib>:"G#Object_EnableDebug.vi"("set (F)"=TRUE, "debug enable (F)"=w684, "error in (no error)"=w687) -> ("error out"=w686:errorcluster)  [unwired: 14 in, 2 out]
        n311 = case shown="True" w684 {
          tunnel: w686 -> [w706 w714]
          tunnel: [w708 w716] -> w690
          tunnel: w692 -> [w707 w715]
          tunnel: w689 -> [w697 w713]
          tunnel: w688 -> [_ w710]
          frame False {
            n312 = Unbundle By Name(w697) -> ("Front Panel"=w696:refnum<vi>)
            n313 = call <vilib>:"G#Debugger_CachedObject.vi"("cached object"=refnum<class "G#Object.lvclass"> refnum, "error in (no error)"=w706, "set"=TRUE) -> ("error out"=w705:errorcluster)  [unwired: 14 in, 2 out]
            n314 = property on="Cached Reference Class Name" class="Str"("Value"="") -> ()  [unwired: 2 in, 2 out]
            n315 = call <vilib>:"GarbageCollector.vi"("error in (no error)"=w705) -> ("error out"=w699:errorcluster)  [unwired: 16 in, 2 out]
            n316 = property on="CachedObjId" class="DigNum (strict)"("Value"=u32 0 ("CachedObjId")) -> ()  [unwired: 2 in, 2 out]
            n317 = call "Empty Picture"() -> ("empty picture"=w700:picture)
            n318 = invoke on="Method VI Panel" class="SubPanel" method="Remove VI"(error in=w699) -> (error out=w698:errorcluster)  [unwired: 2 in, 2 out]
            n319 = property on="Icon" class="Pict"("Value"=w700) -> ()  [unwired: 2 in, 2 out]
            n320 = call <vilib>:"G#Debugger_ClearTree.vi"("Front Panel"=w696, "Tree"=w707, "error in (no error)"=w698) -> ("error out"=w708:errorcluster)  [unwired: 16 in]
          }
          frame True {
            n321 = Unbundle By Name(w713) -> ("Front Panel"=w709:refnum<vi>, "Active Project"=w712:refnum<vi>)
            n322 = Not A Number/Path/Refnum?(number/path/refnum=w712) -> (NaN/Path/Refnum?=w711:bool)
            n323 = case shown="False" w711 {
              tunnel: [w722 w726] -> w716
              tunnel: w715 -> [w721 _]
              tunnel: w714 -> [w719 w726]
              tunnel: w712 -> [w718 _]
              tunnel: w710 -> [_ w725]
              tunnel: w709 -> [w717 _]
              frame False {
                n324 = call <vilib>:"G#Object_StartExternalCreateProcess.vi"("error in (no error)"=w719) -> ("error out"=w720:errorcluster)  [unwired: 18 in]
                n325 = call <vilib>:"G#Debugger_PopulateActiveDebugTree.vi"("Front Panel"=w717, "Tree"=w721, "Active Project"=w718, "error in (no error)"=w720) -> ("error out"=w722:errorcluster)  [unwired: 15 in]
              }
              frame True {
                (unwired) "%s not valid anymore!"
                n326 = Format Into String(w725) -> (resulting string=w724:string)  [unwired: 3 in, 1 out]
                n327 = property on="Enable Active Debug" class="Bool (strict)"("Value"=FALSE ("Enable Active Debug")) -> ()  [unwired: 2 in, 2 out]
                n328 = One Button Dialog(message=w724) -> ()  [unwired: 1 in, 1 out]
              }
            }
          }
        }
      }
      event "Window Transparency": Value Change {
        n329 = event-data() -> ()  [unwired: 1 in, 5 out]
        n330 = control-ref of="This VI"() -> (w731:refnum<vi>)
        n331 = Not Equal To 0?(x="Window Transparency") -> (x != 0?=w727:bool)
        n332 = property class="VI"(reference=w731, error in=w730, "FP:Transparency"="Window Transparency", "FP:RunTransparently"=w727) -> (error out=w729:errorcluster)  [unwired: 1 out]
      }
      event "Window Behaviour": Value Change {
        n333 = event-data() -> ()  [unwired: 1 in, 5 out]
        n334 = Select(t=T4."Floating" ("Front Panel Window:Behavior"), s="Window Behaviour", f=T4."Default" ("Front Panel Window:Behavior")) -> (s? t:f=w732:T4)
        n335 = property class="VI"(error in=w737, "FP.Behavior"=w732) -> (error out=w736:errorcluster)  [unwired: 1 in, 1 out]
      }
      event "External Create Process Running": Value Change {
        n336 = event-data() -> ()  [unwired: 1 in, 5 out]
        n337 = case shown="False" "External Create Process Running" {
          tunnel: w740 -> [w742 w744]
          tunnel: [w741 w743] -> w739
          frame False {
            n338 = call <vilib>:"G#Object_StopExternalCreateProcess.vi"("error in (no error)"=w742) -> ("error out"=w741:errorcluster)  [unwired: 17 in, 1 out]
          }
          frame True {
            n339 = call <vilib>:"G#Object_StartExternalCreateProcess.vi"("error in (no error)"=w744) -> ("error out"=w743:errorcluster)  [unwired: 18 in]
          }
        }
      }
      event "Help": Value Change {
        n340 = event-data() -> ()  [unwired: 1 in, 5 out]
        n341 = property class="App"() -> ("OS.Name"=w745:string, "OS.Version"=w746:string)  [unwired: 2 in, 2 out]
        n342 = case shown="\"Windows\"..\"Windowt\"" w745 {
          tunnel: w746 -> [_ _]
          frame Default {
            n343 = call-poly <vilib>:"Open URL in Default Browser.vi"("URL"="http://www.addq.se/document/GsharpOnlineManual.htm" ("message")) -> ()  [unwired: 5 in, 2 out]
          }
          frame "Windows".."Windowt" {
            w756 = TRUE  # run minimized? (F)
            w757 = FALSE  # wait until completion? (T)
            n344 = VI Library() -> (path=w755:path)
            n345 = Strip Path(path=w755) -> (stripped path=w754:path)  [unwired: 1 out]
            n346 = Build Path(base path=w754, name or relative path="help") -> (appended path=w752:path)
            n347 = Build Path(base path=w752, name or relative path="_AddQ") -> (appended path=w750:path)
            n348 = call <vilib>:"System Exec.vi"("run minimized? (F)"=w756, "wait until completion? (T)"=w757, "working directory"=w750, "command line"="cmd /c hh.exe \"Gsharp.chm::GsharpDebugger.htm\"") -> ()  [unwired: 4 in, 4 out]
          }
        }
      }
      event "Filter Expression": Value Change {
        n349 = event-data() -> ("NewVal"=w759:string)  [unwired: 1 in, 4 out]
        n350 = Format Into String(format string="Changed filter expression to '%s'!" ("text"), w759) -> (resulting string=w758:string)  [unwired: 2 in, 1 out]
        n351 = call <vilib>:"G#Object_SendUserEvent.vi"("text"=w758, "error in (no error)"=w762) -> ("error out"=w761:errorcluster)  [unwired: 16 in, 1 out]
      }
      event "Highlight Aggregates?": Value Change {
        n352 = event-data() -> ("NewVal"=w765:bool)  [unwired: 1 in, 4 out]
        n353 = case shown="False" w765 {
          tunnel: w767 -> [w775 w778]
          tunnel: w766 -> [w774 _]
          tunnel: [w770 w779] -> w764
          tunnel: w763 -> [w769 w777]
          frame False {
            # "redraw FP"
            n354 = call <vilib>:"G#Debugger_Highlight.vi"("Tree"=w774, "error in (no error)"=w775) -> ("error out"=w771:errorcluster)  [unwired: 17 in]
            n355 = Unbundle By Name(w769) -> ("Front Panel"=w768:refnum<vi>)
            n356 = property class="Pnl"(reference=w768, error in=w771, "DeferPanUpdts"=FALSE ("Defer Panel Updates"), "DeferPanUpdts"=TRUE ("Defer Panel Updates")) -> (error out=w770:errorcluster)  [unwired: 1 out]
          }
          frame True {
            n357 = Unbundle By Name(w777) -> ("GUI event"=w776:refnum<user-event>)
            n358 = Generate User Event(user event=w776, event data cluster="Highlight aggregates" ("event data"), error in=w778) -> (error out=w779:errorcluster)  [unwired: 1 in, 1 out]
          }
        }
      }
      event "Connect": Value Change {
        n359 = event-data() -> ()  [unwired: 1 in, 5 out]
        n360 = call <vilib>:"StopDebugClient.vi"("error in (no error)"=w788) -> ("error out"=w783:errorcluster)  [unwired: 18 in]
        n361 = property on="Connected?" class="Bool (strict)"(error in=w783, "Value"=FALSE ("Connected?")) -> (error out=w782:errorcluster)  [unwired: 1 in, 1 out]
        n362 = call <vilib>:"Dialog_SelectTarget.vi"("error in (no error)"=w782) -> ("target address out"=w790:string, "cancel?"=w789:bool, "TCP port out"=w785:u16, "error out"=w791:errorcluster)  [unwired: 15 in]
        n363 = case shown="False" w789 {
          tunnel: w791 -> [w795 w796]
          tunnel: w790 -> [w794 _]
          tunnel: [w793 w796] -> w787
          tunnel: w785 -> [w792 _]
          frame False {
            n364 = call <vilib>:"StartDebugClient.vi"("target address"=w794, "TCP port"=w792, "error in (no error)"=w795) -> ("error out"=w793:errorcluster)  [unwired: 16 in]
          }
          frame True {
          }
        }
        n365 = property on="Poll Time (ms)" class="DigNum (strict)"(error in=w787, "Value"=1000 ("Poll time (ms)")) -> (error out=w784:errorcluster)  [unwired: 1 in, 1 out]
      }
      event "OpClnUI": Value Change {
        n366 = event-data() -> ()  [unwired: 1 in, 1 out]
        n367 = property on="RootClass" class="Ring (strict)"(error in=w813) -> (error out=w801:errorcluster, "Strings []"=w812:string[], "Value"=w811:i32)  [unwired: 1 in, 1 out]
        n368 = Index Array(array=w812, index=w811) -> (element=w805:string)
        n369 = vi-ref "G#Debugger.lvlib:G#Debugger_CloneUI.vi"() -> (w809:refnum<vi>)
        n370 = property class="VI"(reference=w809, error in=w801) -> (reference out=w804:refnum<vi>, error out=w799:errorcluster, "Path"=w808:path)
        n371 = Open VI Reference(type specifier VI Refnum (for type only)=refnum<vi> refnum, vi path=w808, options=128, error in (no error)=w799) -> (vi reference=w806:refnum<vi>, error out=w810:errorcluster)  [unwired: 2 in]
        n372 = call-by-ref "Start Asynchronous Call"(reference=w806, error in=w810, "RootClass"=w805) -> (reference out=w803:refnum<vi>, error out=w802:errorcluster)  [unwired: 19 in]
        n373 = Close Reference(reference=w803, error in (no error)=w802) -> (error out=w800:errorcluster)
        n374 = Close Reference(reference=w804, error in (no error)=w800) -> (error out=w798:errorcluster)
      }
    }
    n375 = call <vilib>:"G#Debugger_CheckError.vi"("refs"=w32, "error in (no error)"=w33) -> ("error out"=w34:errorcluster)  [unwired: 17 in]
  }
  n376 = while {
    shift-right: [w835] -> w15
    shift-left: w6 -> [w821]
    tunnel: w21 -> [w815]
    shift-right: [w832] -> w13
    shift-left: _ -> [w820]
    tunnel: w12 -> [w831]
    stop <- w833 stop-if-true
    w822 = TRUE  # create if needed
    # "G# event processing loop"
    n377 = Unbundle By Name(w815) -> ("GUI event"=w817:refnum<user-event>, "class information dvr"=w816:refnum<data-value>)
    n378 = Unbundle By Name(w815) -> ("Front Panel"=w814:refnum<vi>)
    n379 = call <vilib>:"G#Object_GetEvent.vi"("create if needed (T)"=w822, "error in (no error)"=w821) -> ("G# event"=w828:refnum<user-event>, "created new"=w827:bool, "error out"=w823:errorcluster)  [unwired: 13 in, 2 out]
    n380 = feedback #3() -> (w829:refnum<user-event>)  [unwired: 1 in]
    n381 = feedback-in #3(w828) -> ()
    n382 = Not A Number/Path/Refnum?(number/path/refnum=w820) -> (NaN/Path/Refnum?=w824:bool)
    n383 = Not Equal?(x=w828, y=w829) -> (x != y?=w826:bool)
    n384 = Compound Arithmetic op=OR(w826, w824, w827) -> (w825:bool)
    n385 = case shown="True" w825 {
      tunnel: w823 -> [w837 w847]
      tunnel: w820 -> [w836 w845]
      tunnel: [w837 w841] -> w818
      tunnel: w828 -> [_ w843]
      tunnel: [w836 w842] -> w819
      tunnel: w817 -> [_ w838]
      frame False {
      }
      frame True {
        n386 = Not A Number/Path/Refnum?(number/path/refnum=w845) -> (NaN/Path/Refnum?=w846:bool)
        n387 = case shown="False" w846 {
          tunnel: w847 -> [w849 w851]
          tunnel: [w850 w851] -> w844
          tunnel: w845 -> [w848 _]
          frame False {
            n388 = Unregister For Events(event registration refnum=w848, error in=w849) -> (error out=w850:errorcluster)
          }
          frame True {
          }
        }
        n389 = register-events(error in=w844, w843, w838) -> (reference out=w842:refnum<event-registration>, error out=w839:errorcluster)  [unwired: 1 in]
        n390 = Generate User Event(user event=w838, event data cluster="Refresh" ("event data"), error in=w839) -> (error out=w841:errorcluster)  [unwired: 1 in, 1 out]
      }
    }
    n391 = event shown="[2] <G# event>: User Event" {
      selector: w819 -> [_ _ _ _ _]
      dyn-events: [_ _ _ _ _] -> w832
      timeout: 100 -> [_ _ _ _ _]
      tunnel: w818 -> [w853 w857 w888 w977 w998]
      tunnel: [w852 w856 w866 w975 w997] -> w834
      tunnel: [_ w855 _ _ _] -> w833
      tunnel: w831 -> [_ _ w886 _ _]
      tunnel: w817 -> [_ _ w864 _ _]
      tunnel: w816 -> [_ _ w863 _ _]
      tunnel: w814 -> [_ _ w862 _ _]
      event Timeout {
        n392 = event-data() -> ()  [unwired: 1 in, 2 out]
        n393 = call <vilib>:"G#Object_IsExternalCreateProcessRunning.vi"("error in (no error)"=w853) -> ("external create process running?"=w854:bool, "error out"=w852:errorcluster)  [unwired: 15 in, 2 out]
        n394 = property on="External Create Process Running" class="Bool (strict)"("Value"=w854) -> ()  [unwired: 2 in, 2 out]
      }
      event User Event {
        n395 = event-data() -> ("GUI event"=w858:string)  [unwired: 1 in, 3 out]
        n396 = case shown="\"Exit\"" w858 {
          tunnel: w857 -> [w859 w861]
          tunnel: [w859 w861] -> w856
          tunnel: [_ TRUE] -> w855
          frame Default {
          }
          frame "Exit" {
          }
        }
      }
      event User Event {
        n397 = event-data() -> ("Time Stamp"=w882:timestamp, "LogText"=w879:string, "EventType"=w889:T10, "ObjectInfo"=w887:T11, "Ref"=w880:refnum<class "G#Object.lvclass">, "Parameters"=w878:variant[])  [unwired: 1 in]
        n398 = Format Date/Time String(time format string (%c)="%H:%M:%S%3u", seconds (now)=w882) -> (date/time string=w881:string)  [unwired: 1 in]
        n399 = case shown="\"Looked up existing\"" w889 {
          tunnel: w888 -> [w910 w911 w922 w948 w961]
          tunnel: [w910 w913 w918 w943 w960] -> w866
          tunnel: w887 -> [_ _ w920 w947 _]
          tunnel: w864 -> [_ w912 w916 _ w959]
          tunnel: w863 -> [_ _ w921 w946 _]
          tunnel: w886 -> [_ _ w919 w945 _]
          tunnel: "Tab Control" -> [_ _ w917 w944 w962]
          tunnel: w880 -> [_ _ _ w942 _]
          tunnel: w879 -> [_ _ _ _ _]
          tunnel: w878 -> [_ _ _ _ _]
          tunnel: w862 -> [_ _ w915 w941 _]
          frame Default {
          }
          frame "Garbage collected" {
            n400 = Generate User Event(user event=w912, event data cluster="Clear" ("event data"), error in=w911) -> (error out=w913:errorcluster)  [unwired: 1 in, 1 out]
          }
          frame "Deleted", "Forced delete" {
            n401 = case shown="\"Objects\"" w917 {
              tunnel: w922 -> [w923 w933]
              tunnel: w921 -> [_ w932]
              tunnel: w920 -> [_ w931]
              tunnel: w919 -> [_ w930]
              tunnel: [w923 w926] -> w918
              tunnel: w916 -> [_ w925]
              tunnel: w915 -> [_ w924]
              frame Default {
              }
              frame "Objects" {
                # "Update tree control"
                n402 = call <vilib>:"G#Debugger_RemoveObject.vi"("Objects dvr"=w932, "ObjectInfo"=w931, "error in (no error)"=w933) -> ("Elements"=w935:T13, "error out"=w934:errorcluster)  [unwired: 15 in]
                n403 = property on="Hide Empty Classes?" class="Bool (strict)"() -> ("Value"=w929:bool)  [unwired: 2 in, 2 out]
                n404 = call <vilib>:"G#Debugger_RemoveObjectFromTree.vi"("Front Panel"=w924, "Tree"=w930, "TreeElement"=w935, "hide empty classes?"=w929, "error in (no error)"=w934) -> ("EmptyTree?"=w927:bool, "error out"=w928:errorcluster)  [unwired: 13 in]
                n405 = case shown="True" w927 {
                  tunnel: w928 -> [w936 w939]
                  tunnel: [w936 w940] -> w926
                  tunnel: w925 -> [_ w938]
                  frame False {
                  }
                  frame True {
                    n406 = Generate User Event(user event=w938, event data cluster="Clear object tab" ("event data"), error in=w939) -> (error out=w940:errorcluster)  [unwired: 1 in, 1 out]
                  }
                }
              }
            }
          }
          frame "Created new" {
            n407 = case shown="\"Objects\"" w944 {
              tunnel: w948 -> [w949 w958]
              tunnel: [w949 w957] -> w943
              tunnel: w947 -> [_ w956]
              tunnel: w946 -> [_ w955]
              tunnel: w945 -> [_ w953]
              tunnel: w942 -> [_ w954]
              tunnel: w941 -> [_ w950]
              frame Default {
              }
              frame "Objects" {
                # "Update tree control"
                n408 = call <vilib>:"G#Debugger_AddObject.vi"("Objects dvr"=w955, "ObjectInfo"=w956, "Ref"=w954, "error in (no error)"=w958) -> ("Elements"=w952:T13[], "error out"=w951:errorcluster)  [unwired: 14 in]
                n409 = call <vilib>:"G#Debugger_AddObjectToTree.vi"("Front Panel"=w950, "Tree"=w953, "Elements"=w952, "error in (no error)"=w951) -> ("error out"=w957:errorcluster)  [unwired: 15 in]
              }
            }
          }
          frame "Looked up existing" {
            n410 = case shown="\"Objects\"" w962 {
              tunnel: w961 -> [w963 w965]
              tunnel: [w963 w966] -> w960
              tunnel: w959 -> [_ w964]
              frame Default {
              }
              frame "Objects" {
                n411 = Generate User Event(user event=w964, event data cluster="Update attributes" ("event data"), error in=w965) -> (error out=w966:errorcluster)  [unwired: 1 in, 1 out]
              }
            }
          }
        }
        n412 = Concatenate Strings(w881, ": " ("string"), w879) -> (w873:string)
        n413 = To Long Integer(number="Max Lines") -> (32bit integer=w865:i32)
        n414 = case shown="False" "Trace Direction" {
          tunnel: w865 -> [w898 w909]
          tunnel: w873 -> [w895 w906]
          tunnel: [w894 w907] -> w869
          tunnel: "Clear" -> [w893 w905]
          tunnel: string[] [] -> [w890 w902]
          frame False {
            n415 = feedback #4(w890) -> (w892:string[])
            n416 = Select(t=w890, s=w893, f=w892) -> (s? t:f=w891:string[])
            n417 = Build Array (concatenate)(w891, w895) -> (w896:string[])
            n418 = Array Size(array=w896) -> (size(s)=w901:i32)
            n419 = Greater?(x=w901, y=w898) -> (0:w900:bool)
            n420 = Boolean To (0,1)(Boolean=w900) -> (0, 1=w899:i16)
            n421 = To Long Integer(number=w899) -> (32bit integer=w897:i32)
            n422 = Array Subset(array=w896, index=w897, length=w898) -> (w894:string[])
            n423 = feedback-in #4(w894) -> ()
          }
          frame True {
            n424 = feedback #5(w902) -> (w904:string[])
            n425 = Select(t=w902, s=w905, f=w904) -> (s? t:f=w903:string[])
            n426 = Build Array (concatenate)(w906, w903) -> (w908:string[])
            n427 = Array Subset(array=w908, length=w909) -> (w907:string[])  [unwired: 1 in]
            n428 = feedback-in #5(w907) -> ()
          }
        }
        n429 = call <vilib>:"G#Debugger_FilterTrace.vi"("TraceIn"=w869, "FilterExpression"="Filter Expression") -> ("TraceOut"=w868:string[])  [unwired: 17 in]
        n430 = Array To Spreadsheet String(delimiter (Tab)="\r\n", array=w868, 3:"%s" ("format string")) -> (spreadsheet string=→"Trace":string)
      }
      event "Abort VI": Value Change {
        # "This event must be in this loop to be able to abort a running VI"
        n431 = event-data() -> ()  [unwired: 1 in, 1 out]
        n432 = property on="DebugTree" class="Tree (strict)"() -> ("Value"=w968:string)  [unwired: 2 in, 2 out]
        n433 = Match Pattern(string=w968, regular expression="[.][v][i]") -> (before substring=w971:string, match substring=w970:string)  [unwired: 1 in, 2 out]
        n434 = Concatenate Strings(w971, w970) -> (w969:string)
        n435 = String To Path(string=w969) -> (path=w976:path)
        n436 = Open VI Reference(vi path=w976, error in (no error)=w977) -> (vi reference=w974:refnum<vi>, error out=w973:errorcluster)  [unwired: 4 in]
        n437 = case shown="No Error" w973 {
          selector: w973 -> [w978 _]
          tunnel: [w981 errorcluster {"status"=FALSE, "code"=0, "source"=""} ("error out")] -> w975
          tunnel: w974 -> [w979 _]
          frame No Error {
            n438 = property class="VI"(reference=w979, error in=w978) -> (reference out=w982:refnum<vi>, error out=w983:errorcluster, "Exec.State"=w984:T7)
            n439 = case shown="\"Run top level\", \"Running\"" w984 {
              tunnel: w983 -> [w985 w990]
              tunnel: w982 -> [_ w989]
              tunnel: [w985 w987] -> w980
              frame "Bad", Default {
              }
              frame "Run top level", "Running" {
                n440 = invoke class="VI" method="Abort VI"(reference=w989, error in=w990) -> (error out=w988:errorcluster)  [unwired: 1 in, 2 out]
                n441 = property on="Run State" class="Str"("Value"="Aborted!") -> ()  [unwired: 2 in, 2 out]
                n442 = call <vilib>:"Clear Errors.vi"("error in (no error)"=w988) -> ("error out"=w987:errorcluster)  [unwired: 5 in, 1 out]
              }
            }
            n443 = Close Reference(reference=w979, error in (no error)=w980) -> (error out=w981:errorcluster)
          }
          frame Error {
          }
        }
      }
      event "Open Panel": Value Change; "DebugTree": Double Click {
        # "This event must be in this loop to be able to open a running VI"
        n444 = event-data() -> ()  [unwired: 1 in, 4 out]
        n445 = Match Pattern(string="DebugTree", regular expression="[.][v][i]") -> (before substring=w994:string, match substring=w992:string)  [unwired: 1 in, 2 out]
        n446 = Concatenate Strings(w994, w992) -> (w993:string)
        n447 = String To Path(string=w993) -> (path=w1001:path)
        n448 = Open VI Reference(vi path=w1001, error in (no error)=w998) -> (vi reference=w999:refnum<vi>, error out=w1000:errorcluster)  [unwired: 4 in]
        n449 = case shown="No Error" w1000 {
          selector: w1000 -> [w1003 _]
          tunnel: [w1007 errorcluster {"status"=FALSE, "code"=0, "source"=""} ("error in (no error)")] -> w997
          tunnel: w999 -> [w1004 _]
          frame No Error {
            n450 = invoke on="Method VI Panel" class="SubPanel" method="Remove VI"(error in=w1003) -> (error out=w1002:errorcluster)  [unwired: 2 in, 2 out]
            n451 = call <vilib>:"G#Debugger_SetCachedRef.vi"("MethodVIref"=w1004, "error in (no error)"=w1002) -> ("error out"=w1005:errorcluster)  [unwired: 17 in]
            n452 = case shown="No Error" w1005 {
              selector: w1005 -> [w1010 _]
              tunnel: [w1013 errorcluster {"status"=FALSE, "code"=0, "source"=""} ("error out")] -> w1006
              tunnel: w1004 -> [w1012 _]
              frame No Error {
                n453 = vi-ref "G#Debugger.lvlib:G#Debugger_DebugDialog.vi"() -> (w1008:refnum<vi>)
                n454 = invoke on="Method VI Panel" class="SubPanel" method="Insert VI"(error in=w1010, "VI Ref"=w1008) -> (error out=w1009:errorcluster)  [unwired: 2 in, 3 out]
                n455 = call "Empty Picture"() -> ("empty picture"=w1011:picture)
                n456 = property on="Icon" class="Pict"("Value"=w1011) -> ()  [unwired: 2 in, 2 out]
                n457 = property class="VI"(reference=w1012, error in=w1009, "Front Panel.Open"=TRUE ("Front Panel Window:Open")) -> (error out=w1013:errorcluster)  [unwired: 1 out]
              }
              frame Error {
              }
            }
            n458 = Close Reference(reference=w1004, error in (no error)=w1006) -> (error out=w1007:errorcluster)
          }
          frame Error {
          }
        }
      }
    }
    n459 = call <vilib>:"G#Debugger_CheckError.vi"("refs"=w815, "error in (no error)"=w834) -> ("error out"=w835:errorcluster)  [unwired: 17 in]
  }
  n460 = while {
    shift-right: [w1018] -> w5
    shift-left: w6 -> [w1019]
    stop <- TRUE stop-if-true
    # "This thread search for root classes and list. It will exit after."
    n461 = property class="VI"(error in=w1019) -> (error out=w1033:errorcluster, "OwningApp"=w1034:refnum<vi>)  [unwired: 1 in, 1 out]
    n462 = property class="App"(reference=w1034, error in=w1033) -> (reference out=w1032:refnum<vi>, error out=w1026:errorcluster, "Project.OwningProject"=w1027:refnum<vi>)
    n463 = property class="Project"(reference=w1027, error in=w1026) -> (reference out=w1031:refnum<vi>, error out=w1029:errorcluster, "My Computer"=w1030:refnum<vi>)
    n464 = case shown="No Error" w1029 {
      selector: w1029 -> [w1041 w1061]
      tunnel: w1030 -> [w1045 _]
      tunnel: [w1038 w1060] -> w1028
      tunnel: [w1037 _] -> w1036
      frame No Error {
        w1046 = TRUE ("ExcludeDependencies")
        n465 = invoke class="TargetItem" method="Get All Descendents"(reference=w1045, error in=w1041, "Type"="LvClass", "Exclude Dependencies"=w1046, "ExcludeBuilds"=w1046, "ExcludeTargets"=w1046) -> (reference out=w1044:refnum<vi>, error out=w1042:errorcluster, "All Descendents"=w1040:refnum<vi>[])  [unwired: 1 in, 4 out]
        n466 = Close Reference(reference=w1044, error in (no error)=w1042) -> (error out=w1043:errorcluster)
        n467 = for {
          tunnel: w1040 -> [w1058] mode=indexing
          shift-right: [w1048] -> w1039
          shift-left: w1043 -> [w1059]
          tunnel: [w1050] -> w1037 mode=indexing if=w1049
          w1057 = refnum<vi> refnum  # LVClassLibrary
          n468 = To More Specific Class(target class=w1057, reference=w1058, error in=w1059) -> (specific class reference=w1051:refnum<vi>, error out=w1052:errorcluster)
          n469 = property class="LVClassLibrary"(reference=w1051, error in=w1052) -> (error out=w1048:errorcluster, "Name"=w1055:string)  [unwired: 1 out]
          n470 = Match Pattern(string=w1055, regular expression="G#Object" ("string")) -> (offset past match=w1056:i32)  [unwired: 1 in, 3 out]
          n471 = Match Pattern(string=w1055, regular expression=".lvclass") -> (before substring=w1050:string)  [unwired: 1 in, 3 out]
          n472 = Greater Or Equal To 0?(x=w1056) -> (x >= 0?=w1049:bool)
        }
        n473 = Close Reference(reference=w1040, error in (no error)=w1039) -> (error out=w1038:errorcluster)
      }
      frame Error {
        n474 = call <vilib>:"Clear Errors.vi"("error in (no error)"=w1061) -> ("error out"=w1060:errorcluster)  [unwired: 5 in, 1 out]
      }
    }
    n475 = Close Reference(reference=w1031, error in (no error)=w1028) -> (error out=w1025:errorcluster)
    n476 = Close Reference(reference=w1032, error in (no error)=w1025) -> (error out=w1024:errorcluster)
    n477 = Empty Array?(array=w1036) -> (empty?=w1023:bool)
    n478 = Not(x=w1023) -> (.not. x?=w1035:bool)
    n479 = call <vilib>:"Clear Errors.vi"("error in (no error)"=w1024) -> ("error out"=w1021:errorcluster)  [unwired: 5 in, 1 out]
    n480 = property on="RootClass" class="Ring (strict)"(error in=w1021, "Strings []"=w1036, "Visible"=w1035, "Value"=0) -> (error out=w1022:errorcluster)  [unwired: 1 in, 1 out]
    n481 = property on="OpClnUI" class="Bool"(error in=w1022, "Visible"=w1035) -> (error out=w1018:errorcluster)  [unwired: 1 in, 1 out]
  }
  n482 = Unregister For Events(event registration refnum=w13, error in=w15) -> (error out=w14:errorcluster)
  n483 = Unregister For Events(event registration refnum=w17, error in=w18) -> (error out=w16:errorcluster)
  n484 = Merge Errors(w16, w14, w5) -> (w20:errorcluster)
  n485 = call <vilib>:"G#Debugger_Close.vi"("refs"=w21, "error in (no error)"=w20) -> ("error out"=w7:errorcluster)  [unwired: 17 in]
  n486 = case shown="No Error" w7 {
    selector: w7 -> [w1062 w1064]
    tunnel: [w1062 _] -> w8
    frame No Error {
    }
    frame Error {
      n487 = Unbundle By Name(w1064) -> ("source"=w1063:string)
      n488 = One Button Dialog(message=w1063) -> ()  [unwired: 1 in, 1 out]
    }
  }
  n489 = invoke class="VI" method="FP.Close"(error in=w8) -> ()  [unwired: 2 in, 3 out]
